vi "Creer un profil EUROTHERM EPC3000.vi"() -> ()   [LabVIEW 2022 SP3]
uses:
  Enum/Enum r15.ctl
  <vilib>/Utility/miscctls.llb/LVDateTimeRec.ctl
  Variables globales/Variable glob generale.vi
  Variables globales/Variables glob EUROTHERM.vi
panel:
  out "Programme 10":cluster{"chaîne":string, "Valeur":dbl}[][](array[cluster]) {"Valeur" format="%#.2f"}
  out "Programme 9":cluster{"chaîne":string, "Valeur":dbl}[][](array[cluster]) {"Valeur" format="%#.2f"}
  out "Programme 8":cluster{"chaîne":string, "Valeur":dbl}[][](array[cluster]) {"Valeur" format="%#.2f"}
  out "Programme 7":cluster{"chaîne":string, "Valeur":dbl}[][](array[cluster]) {"Valeur" format="%#.2f"}
  out "Programme 6":cluster{"chaîne":string, "Valeur":dbl}[][](array[cluster]) {"Valeur" format="%#.2f"}
  out "Programme 5":cluster{"chaîne":string, "Valeur":dbl}[][](array[cluster]) {"Valeur" format="%#.2f"}
  out "référence en sortie":refnum<vi>
  out "Programme 1":cluster{"chaîne":string, "Valeur":dbl}[][](array[cluster]) {"Valeur" format="%#.2f"}
  in  "Insérer segment":bool
  in  "Segment à éditer/supprimer":u8=1 max=26 step=1
  in  "Supprimer segment":bool
  in  "Modif seg":bool
  in  "Charger":bool
  in  "Sauvegarder":bool
  in  "Début du profil":timestamp format="%<%H:%M:%S\n%A %d/%m/%y>T"
  in  "Onglet_Tinit":enum32{"Définir Tinit", "Acquérir Tinit"}(tab)
  in  "Val_Tinit":dbl caption="Valeur initiale. (°C)" format="%.1f"
  in  "Num_reg":u8=1 caption="Adresse régulateur" max=3
  in  "COM régulateur":u16(ring) items=["COM2"]
  in  "Ajouter données":bool
  in  "Ajouter segment":bool
  in  "stop":bool
  in  "Visualiser le profil":bool
  in  "A2":bool
  in  "A1":bool
  in  "Palier":bool
  in  "RT":bool
  in  "RV":bool
  in  "Fin":bool
  in  "Appel":bool
  in  "Saut":bool
  out "Profil":cluster{"Y":dbl[], "Y":dbl[]}[](graph)
  out "Type de fin":string
  in  "Alarme haute":dbl caption="Alarme haute (°C)" min=-199.9 max=300.0 format="%#.1f"
  in  "Alarme basse":dbl caption="Alarme basse (°C)" min=-199.9 max=300.0 format="%#.1f"
  out "Indicateur_Données à éditer":bool
  in  "Comm_Unité de palier":u16(ring) caption="Unité de palier" items=["Seconde(s)", "Minute(s)", "Heure(s)"]
  in  "Comm_Unité de rampe":u16(ring) caption="Unité de rampe" items=["Seconde(s)", "Minute(s)", "Heure(s)"]
  out "Configuration":cluster{"Command (PV)":string, dbl}[](array[cluster]) {"?" format="%#.2f"}
  out "Programme 4":cluster{"chaîne":string, "Valeur":dbl}[][](array[cluster]) {"Valeur" format="%#.2f"}
  out "Programme 3":cluster{"chaîne":string, "Valeur":dbl}[][](array[cluster]) {"Valeur" format="%#.2f"}
  out "Programme 2":cluster{"chaîne":string, "Valeur":dbl}[][](array[cluster]) {"Valeur" format="%#.2f"}
  in  "Onglets_programmes":T1(tab)
  out "Listing programme 1":string
  out "Listing programme 2":string
  out "Listing programme 3":string
  out "Listing programme 4":string
  out "Listing programme 5":string
  out "Listing programme 6":string
  out "Listing programme 7":string
  out "Listing programme 8":string
  out "Listing programme 9":string
  out "Listing programme 10":string
  in  "Onglet_segments":T2(tab)
  in  "Type de fin":u8(ring) items=["Palier"]
  in  "Pente rampe vitesse":sgl min=0 format="%.1g"
  in  "Cible rampe vitesse":dbl caption="Cible rampe vitesse (°C)" min=-199.9 max=300.0 format="%.1f"
  out "Indicateur_Unité de rampe 2":string
  out "Indicateur_Unité de rampe 1":string
  in  "Durée rampe temps":sgl min=0 format="%.1g"
  in  "Cible rampe temps":dbl caption="Cible rampe temps (°C)" min=-199.9 max=300.0 format="%.1f"
  in  "Durée palier":sgl min=0 format="%.1f"
  out "Indicateur_Unité de palier":string
  in  "Cible saut (°C)":dbl min=-199.9 max=300.0 format="%#.1f"
  in  "Nb cycles":u8 caption="Nombre de cycles"
  in  "Numéro prog":u8=1 caption="Numéro de programme" min=1 max=10
  # "création d'un fichier\ncontenant le profil de régulation EPC3000"
  # "Indice seg.:"
  # "Ce logiciel et les informations qu'il contient, sont la propriété de l’IAS et ne peuvent être diffusés sans l’autorisation de la Station d’étalonnage"
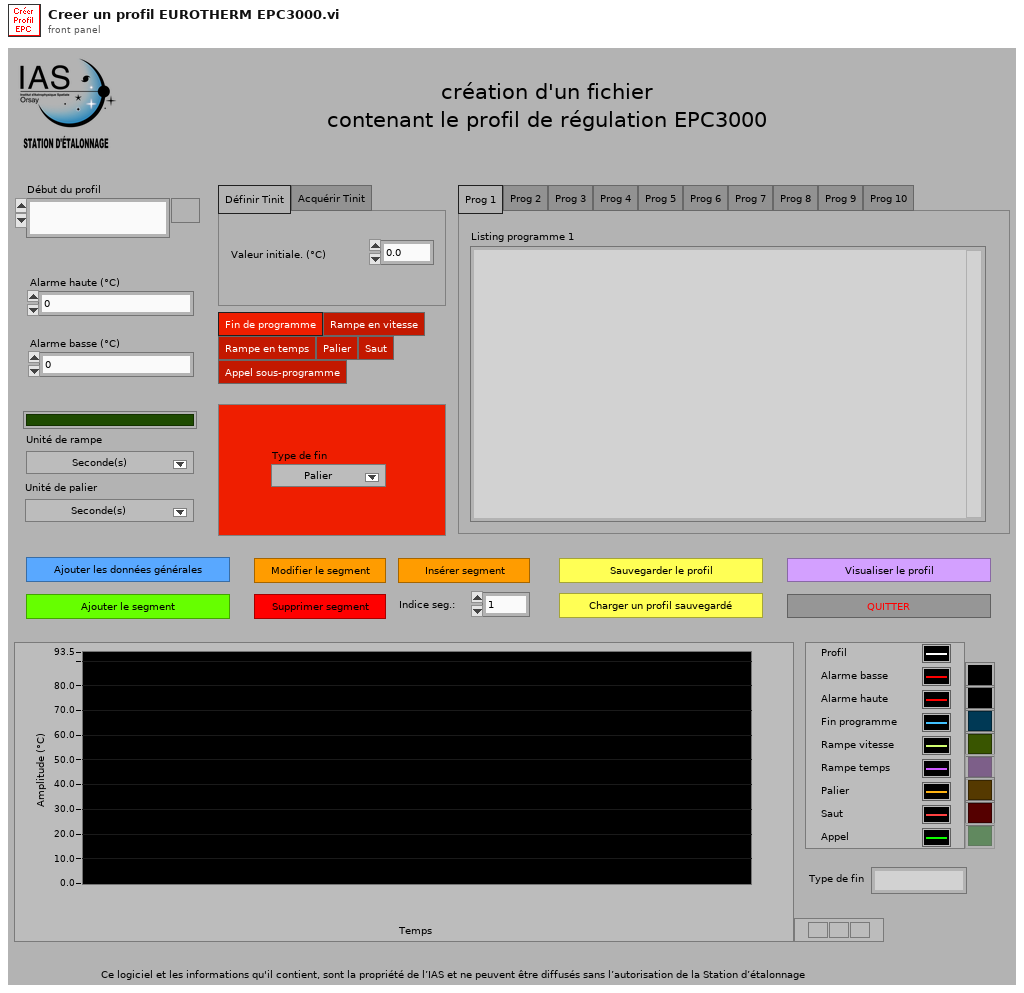
[diagram p1: front panel]
types:
  T1 = enum32{"Prog 1", "Prog 2", "Prog 3", "Prog 4", "Prog 5", "Prog 6", "Prog 7", "Prog 8", "Prog 9", "Prog 10"}
  T2 = enum32{"Fin de programme", "Rampe en vitesse", "Rampe en temps", "Palier", "Saut", "Appel sous-programme"}
  T3 = enum32{"Invalid", "Standard", "Closed", "Hidden", "Minimized", "Maximized"}
  T4 = typedef "Enum r15.ctl" = enum16{"init", "ouvrir fichier", "config", "prog 1", "prog 2", "prog 3", "prog 4", "prog 5", "prog 6", "prog 7", "prog 8", "prog 9", "prog 10", "fin"}
  T5 = cluster{"config":cluster{"key":string, "value":dbl}[], "Prog 1":cluster{string, dbl}[][], "Prog 2":cluster{string, dbl}[][], "Prog 3":cluster{string, dbl}[][], "Prog 4":cluster{string, dbl}[][], "Prog 5":cluster{string, dbl}[][], "Prog 6":cluster{string, dbl}[][], "Prog 7":cluster{string, dbl}[][], "Prog 8":cluster{string, dbl}[][], "Prog 9":cluster{string, dbl}[][], "Prog 10":cluster{string, dbl}[][]}
  T6 = typedef "LVDateTimeRec.ctl" = cluster{"fractional second":dbl, "second":i32, "minute":i32, "hour":i32, "day of month":i32, "month":i32, "year":i32, "day of week":i32, "day of year":i32, "DST":i32}
  T7 = cluster{"chaîne o":string, "Received Value":dbl}[][]
  T8 = cluster{"Configuration":cluster{"Command (PV)":string, dbl}[], "Programme_sortie":cluster{"chaîne":string, "Valeur":dbl}[][], "Programme_sortie":cluster{"chaîne":string, "Valeur":dbl}[][], "Programme_sortie":cluster{"chaîne":string, "Valeur":dbl}[][], "Programme_sortie":cluster{"chaîne":string, "Valeur":dbl}[][], "Programme_sortie":cluster{"chaîne":string, "Valeur":dbl}[][], "Programme_sortie":cluster{"chaîne":string, "Valeur":dbl}[][], "Programme_sortie":cluster{"chaîne":string, "Valeur":dbl}[][], "Programme_sortie":cluster{"chaîne":string, "Valeur":dbl}[][], "Programme_sortie":cluster{"chaîne":string, "Valeur":dbl}[][], "Programme_sortie":cluster{"chaîne":string, "Valeur":dbl}[][]}
  T9 = enum8{"Enabled", "Disabled", "Disabled and Grayed Out"}
  T10 = cluster{"Configuration":cluster{"Command (PV)":string, dbl}[], "Programme 1":cluster{"chaîne":string, "Valeur":dbl}[][], "Programme 2":cluster{"chaîne":string, "Valeur":dbl}[][], "Programme 3":cluster{"chaîne":string, "Valeur":dbl}[][], "Programme 4":cluster{"chaîne":string, "Valeur":dbl}[][], "Programme 5":cluster{"chaîne":string, "Valeur":dbl}[][], "Programme 6":cluster{"chaîne":string, "Valeur":dbl}[][], "Programme 7":cluster{"chaîne":string, "Valeur":dbl}[][], "Programme 8":cluster{"chaîne":string, "Valeur":dbl}[][], "Programme 9":cluster{"chaîne":string, "Valeur":dbl}[][], "Programme 10":cluster{"chaîne":string, "Valeur":dbl}[][]}
  T11 = cluster{"Ev_Saut":dbl[], "Ev_Palier":dbl[], "Ev_Rampe_vitesse":dbl[], "Ev_Rampe_temps":dbl[], "Ev_Appel":dbl[], "Ev_Fin":dbl[], "T_Fin":dbl[], "T_Appel":dbl[], "T_Rampe_temps":dbl[], "T_Rampe_vitesse":dbl[], "T_Palier":dbl[], "T_Saut":dbl[], "Type de fin":string}
  T12 = cluster{"Tempé. max":dbl, "Tempé. min":dbl, "Temps max":dbl, "Temps min":dbl}
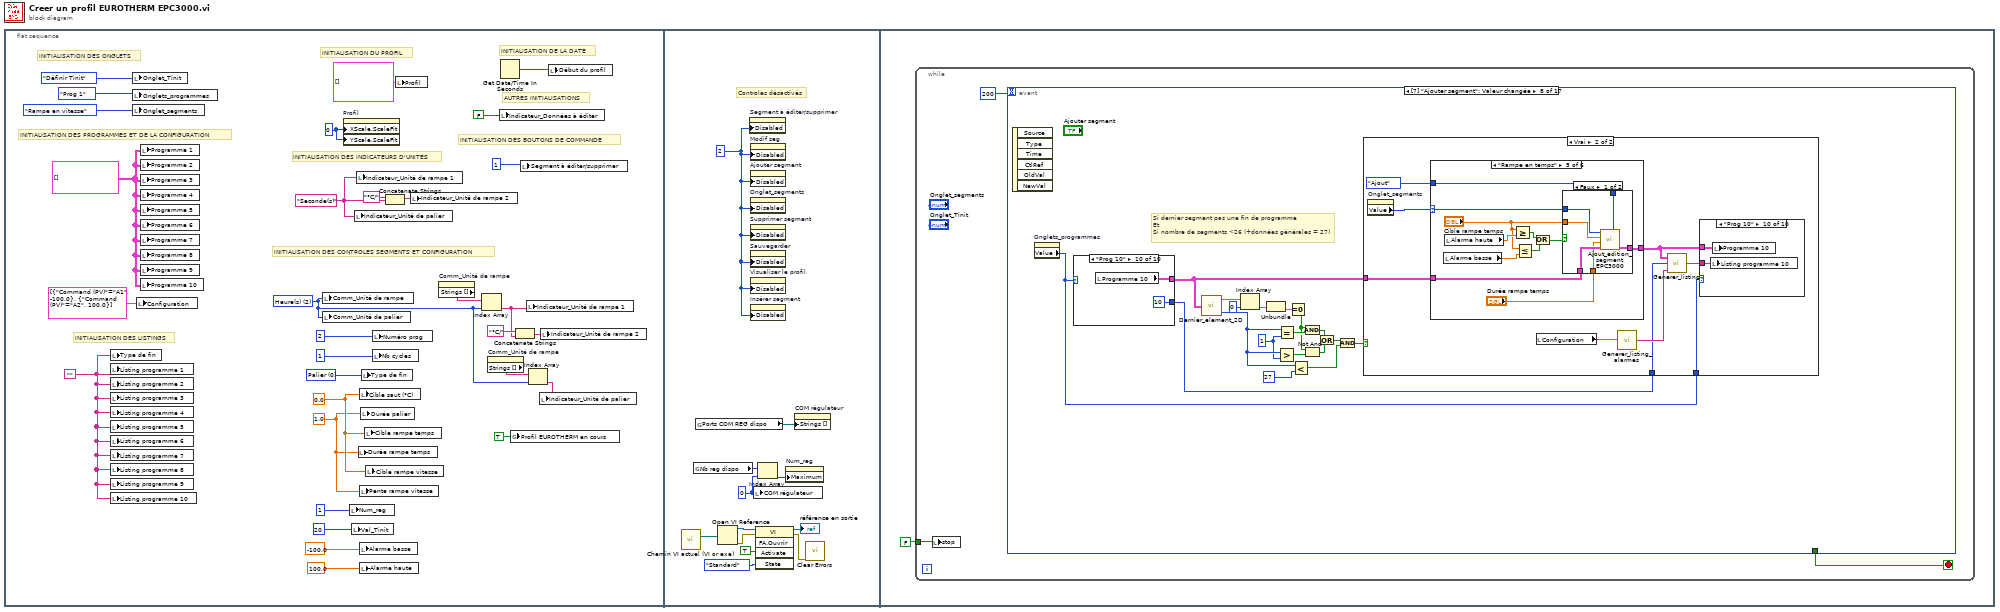
[diagram p0: block diagram]
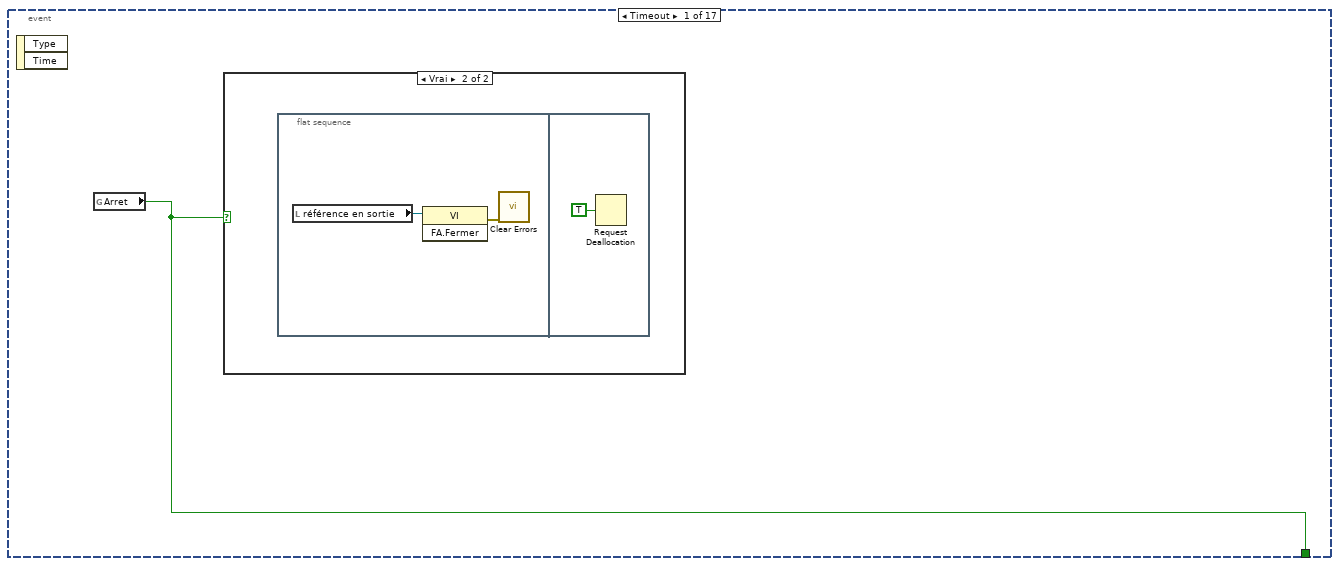
[diagram p2: hidden frame]
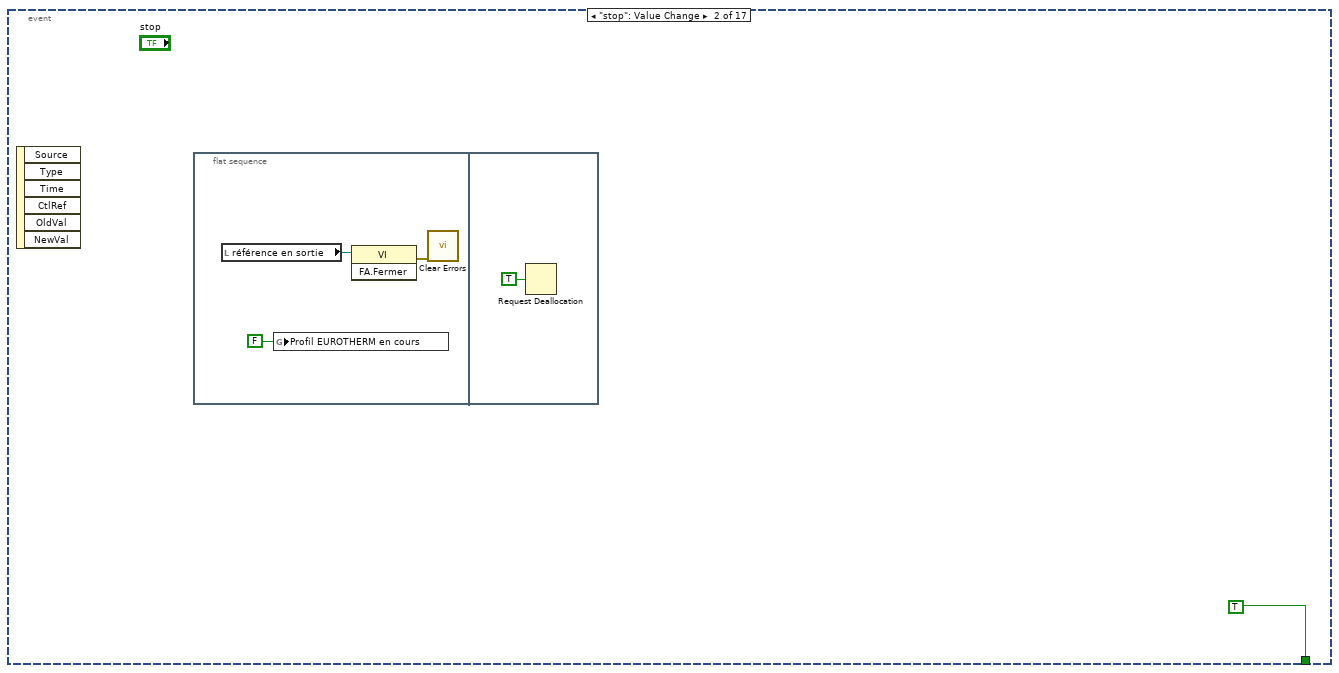
[diagram p4: hidden frame]
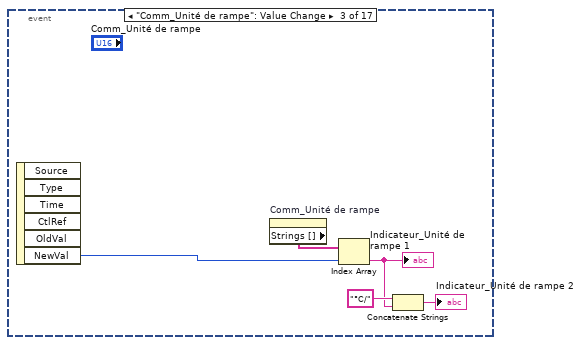
[diagram p5: hidden frame]
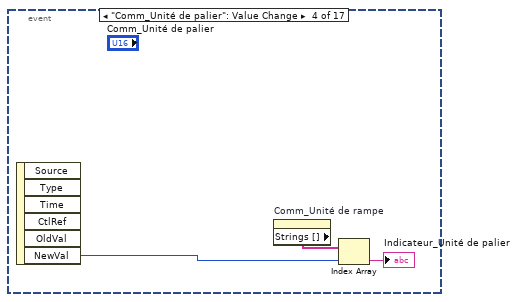
[diagram p6: hidden frame]
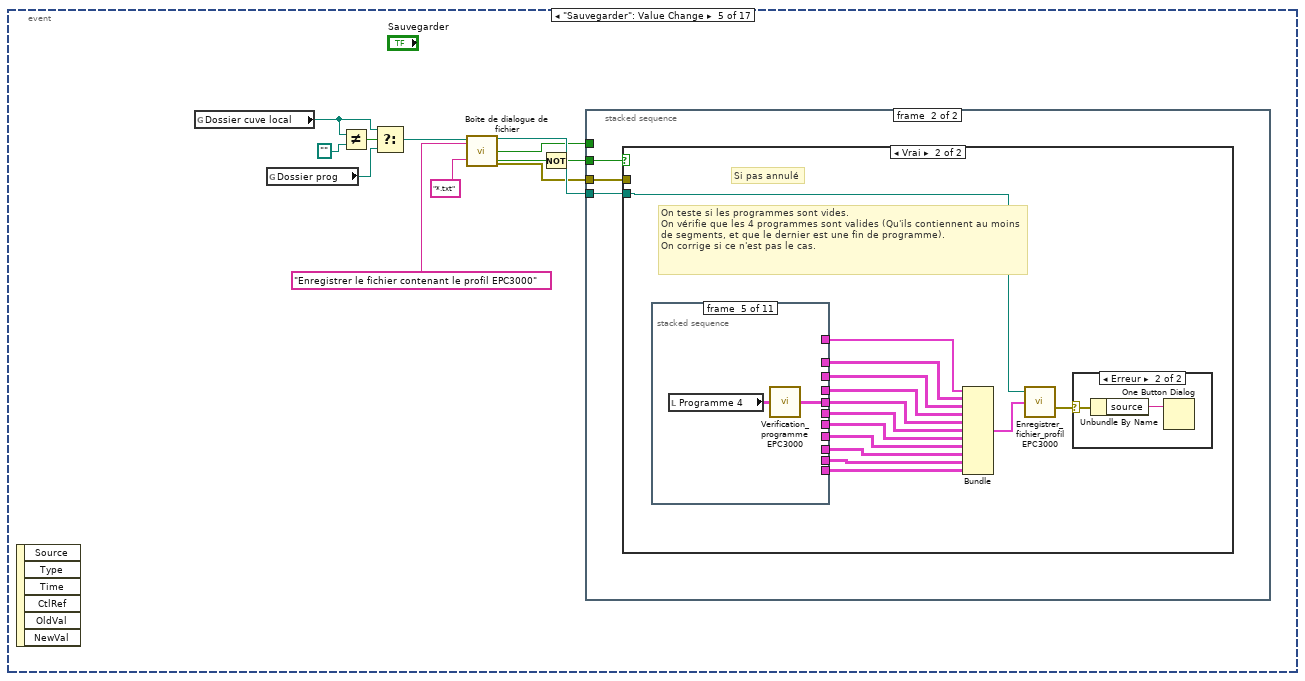
[diagram p7: hidden frame]
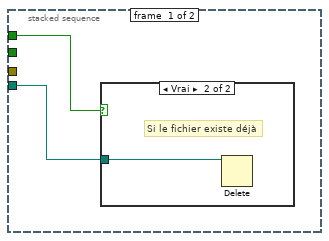
[diagram p8: hidden frame]
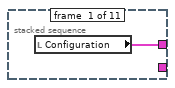
[diagram p11: hidden frame]
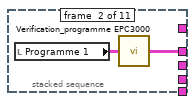
[diagram p12: hidden frame]
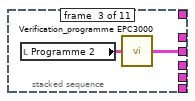
[diagram p13: hidden frame]
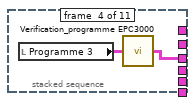
[diagram p14: hidden frame]
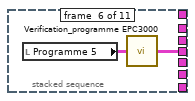
[diagram p15: hidden frame]
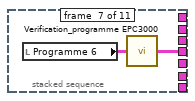
[diagram p16: hidden frame]
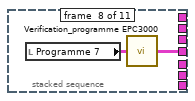
[diagram p17: hidden frame]
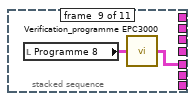
[diagram p18: hidden frame]
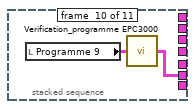
[diagram p19: hidden frame]
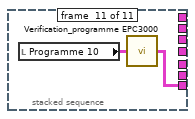
[diagram p20: hidden frame]
diagram:
  n1 = flat-sequence {
    frame #0 {
      w11 = u8 0 items=["Palier"] ("Comm_Type de fin")
      w17 = 1.0 ("Durée rampe temps")
      w18 = 0.0 ("Cible saut (°C)")
      w4 = u16 2 items=["Seconde(s)", "Minute(s)", "Heure(s)"] ("Unité de rampe")
      w23 = u8 0 ("Échelle des X.Ajuster l'échelle")
      w1 = ""
      w2 = T7 [] ("Programme 1")
      w28 = "Seconde(s)" ("Unité de rampe 1")
      # "INITIALISATION DES CONTROLES SEGMENTS ET CONFIGURATION"
      # "AUTRES INITIALISATIONS"
      # "INITIALISATION DES BOUTONS DE COMMANDE"
      # "INITIALISATION DU PROFIL"
      # "INITIALISATION DES LISTINGS"
      # "INITIALISATION DES PROGRAMMES ET DE LA CONFIGURATION"
      # "INITIALISATION DES INDICATEURS D'UNITES"
      # "INITIALISATION DE LA DATE"
      # "INITIALISATION DES ONGLETS"
      n2 = local write "Type de fin"(w1) -> ()
      n3 = local write "Listing programme 1"(w1) -> ()
      n4 = local write "Listing programme 2"(w1) -> ()
      n5 = local write "Listing programme 3"(w1) -> ()
      n6 = local write "Listing programme 4"(w1) -> ()
      n7 = local write "Listing programme 5"(w1) -> ()
      n8 = local write "Listing programme 6"(w1) -> ()
      n9 = local write "Listing programme 7"(w1) -> ()
      n10 = local write "Listing programme 8"(w1) -> ()
      n11 = local write "Listing programme 9"(w1) -> ()
      n12 = local write "Listing programme 10"(w1) -> ()
      n13 = local write "Onglet_Tinit"(enum32{"Définir Tinit", "Acquérir Tinit"}."Définir Tinit" ("Onglet_Tinit")) -> ()
      n14 = local write "Onglets_programmes"(T1."Prog 1" ("Onglets_programmes")) -> ()
      n15 = local write "Onglet_segments"(T2."Rampe en vitesse" ("Commande onglet")) -> ()
      n16 = local write "Configuration"(cluster{"Command (PV)":string, dbl}[] [{"Command (PV)"="A1", -100.0}, {"Command (PV)"="A2", 100.0}] ("Configuration")) -> ()
      n17 = local write "Programme 1"(w2) -> ()
      n18 = local write "Programme 2"(w2) -> ()
      n19 = local write "Programme 3"(w2) -> ()
      n20 = local write "Programme 4"(w2) -> ()
      n21 = local write "Programme 5"(w2) -> ()
      n22 = local write "Programme 6"(w2) -> ()
      n23 = local write "Programme 7"(w2) -> ()
      n24 = local write "Programme 8"(w2) -> ()
      n25 = local write "Programme 9"(w2) -> ()
      n26 = local write "Programme 10"(w2) -> ()
      n27 = local write "Comm_Unité de rampe"(w4) -> ()
      n28 = local write "Comm_Unité de palier"(w4) -> ()
      n29 = property on="Profil" class="GraphXY (strict)"("XScale.ScaleFit"=w23, "YScale.ScaleFit"=w23) -> ()  [unwired: 2 in, 2 out]
      n30 = local write "Num_reg"(u16 1 ("Num_reg")) -> ()
      n31 = local write "Val_Tinit"(u16 20 ("Val_Tinit")) -> ()
      n32 = local write "Indicateur_Unité de palier"(w28) -> ()
      n33 = local write "Indicateur_Unité de rampe 1"(w28) -> ()
      n34 = local write "Durée rampe temps"(w17) -> ()
      n35 = local write "Cible saut (°C)"(w18) -> ()
      n36 = local write "Pente rampe vitesse"(w17) -> ()
      n37 = local write "Alarme basse"(-100.0 ("Comm_Alarme basse")) -> ()
      n38 = local write "Alarme haute"(100.0 ("Comm_Alarme basse")) -> ()
      n39 = local write "Durée palier"(w17) -> ()
      n40 = local write "Type de fin"(w11) -> ()
      n41 = local write "Cible rampe temps"(w18) -> ()
      n42 = local write "Cible rampe vitesse"(w18) -> ()
      n43 = local write "Nb cycles"(u8 1 ("Nombre de cycles")) -> ()
      n44 = local write "Numéro prog"(u8 2 ("Numéro de programme")) -> ()
      n45 = Concatenate Strings("°C/" ("chaîne"), w28) -> (w27:string)
      n46 = local write "Profil"(cluster{"Y":dbl[], "Y":dbl[]}[] [] ("Profil")) -> ()
      n47 = local write "Indicateur_Unité de rampe 2"(w27) -> ()
      n48 = property on="Comm_Unité de rampe" class="MDér (strict)"() -> ("Strings []"=w10:string[])  [unwired: 2 in, 2 out]
      n49 = Index Array(array=w10, index=w4) -> (element=w8:string)
      n50 = property on="Comm_Unité de rampe" class="MDér (strict)"() -> ("Strings []"=w6:string[])  [unwired: 2 in, 2 out]
      n51 = local write "Indicateur_Données à éditer"(FALSE ("Indicateur_Données à éditer")) -> ()
      n52 = Get Date/Time In Seconds() -> (seconds since 1Jan1904=w29:timestamp)
      n53 = global write "Variable glob generale.vi" "Profil EUROTHERM en cours"(TRUE ("Profil en cours")) -> ()
      n54 = Concatenate Strings("°C/" ("chaîne"), w8) -> (w7:string)
      n55 = local write "Segment à éditer/supprimer"(u8 1 ("Segment à éditer")) -> ()
      n56 = local write "Indicateur_Unité de rampe 1"(w8) -> ()
      n57 = Index Array(array=w6, index=w4) -> (element=w5:string)
      n58 = local write "Indicateur_Unité de palier"(w5) -> ()
      n59 = local write "Indicateur_Unité de rampe 2"(w7) -> ()
      n60 = local write "Début du profil"(w29) -> ()
    }
    frame #1 {
      w32 = u16 0
      w43 = u8 2 ("Désactivé")
      # "Controles désactivés"
      n61 = call "Chemin VI actuel (VI or exe).vi"() -> ("Full Path to VI or executable"=w36:path)  [unwired: 14 in, 1 out]
      n62 = global read "Variables glob EUROTHERM.vi" "Nb reg dispo"() -> (w34:u8[])
      n63 = global read "Variables glob EUROTHERM.vi" "Ports COM REG dispo"() -> (w35:refnum<visa-resource-name>[])
      n64 = Open VI Reference(vi path=w36) -> (vi reference=w40:refnum<vi>, error out=w38:errorcluster)  [unwired: 5 in]
      n65 = property on="Segment à éditer/supprimer" class="NumNb (strict)"("Disabled"=w43) -> ()  [unwired: 2 in, 2 out]
      n66 = property on="Modif seg" class="Bool"("Disabled"=w43) -> ()  [unwired: 2 in, 2 out]
      n67 = property on="Ajouter segment" class="Bool"("Disabled"=w43) -> ()  [unwired: 2 in, 2 out]
      n68 = property on="Onglet_segments" class="Onglet (strict)"("Disabled"=w43) -> ()  [unwired: 2 in, 2 out]
      n69 = property on="Supprimer segment" class="Bool"("Disabled"=w43) -> ()  [unwired: 2 in, 2 out]
      n70 = property on="Sauvegarder" class="Bool"("Disabled"=w43) -> ()  [unwired: 2 in, 2 out]
      n71 = property on="Visualiser le profil" class="Bool"("Disabled"=w43) -> ()  [unwired: 2 in, 2 out]
      n72 = property on="Insérer segment" class="Bool"("Disabled"=w43) -> ()  [unwired: 2 in, 2 out]
      n73 = local write "COM régulateur"(w32) -> ()
      n74 = invoke class="VI" method="FA.Ouvrir"(reference=w40, error in=w38, "Activate"=TRUE ("Activer ?"), "State"=T3."Standard" ("État")) -> (reference out=→"référence en sortie":refnum<vi>, error out=w37:errorcluster)  [unwired: 1 in, 3 out]
      n75 = Index Array(array=w34, index=w32) -> (element=w33:u8)
      n76 = property on="Num_reg" class="NumNb (strict)"("Maximum"=w33) -> ()  [unwired: 2 in, 2 out]
      n77 = property on="COM régulateur" class="MDér (strict)"("Strings []"=w35) -> ()  [unwired: 2 in, 2 out]
      n78 = call <vilib>:"Clear Errors.vi"("error in (no error)"=w37) -> ()  [unwired: 5 in, 2 out]
    }
    frame #2 {
      n79 = while {
        tunnel: FALSE ("stop") -> [w46]
        stop <- w47 stop-if-true
        n80 = local write "stop"(w46) -> ()
        n81 = event shown="[7] \"Ajouter segment\": Valeur changée" {
          selector: _ -> [_ _ _ _ _ _ _ _ _ _ _ _ _ _ _ _ _]
          dyn-events: _ -> [_ _ _ _ _ _ _ _ _ _ _ _ _ _ _ _ _]
          timeout: 200 -> [_ _ _ _ _ _ _ _ _ _ _ _ _ _ _ _ _]
          tunnel: [w48 TRUE ("stop") _ _ _ _ _ _ _ _ _ _ _ _ _ _ _] -> w47
          event Timeout {
            n82 = event-data() -> ()  [unwired: 1 in, 2 out]
            n83 = global read "Variable glob generale.vi" "Arret"() -> (w48:bool)
            n84 = case shown="Vrai" w48 {
              frame False {
              }
              frame True {
                n85 = flat-sequence {
                  frame #0 {
                    n86 = local read "référence en sortie"() -> (w49:refnum<vi>)
                    n87 = invoke class="VI" method="FA.Fermer"(reference=w49) -> (error out=w50:errorcluster)  [unwired: 2 in, 2 out]
                    n88 = call <vilib>:"Clear Errors.vi"("error in (no error)"=w50) -> ()  [unwired: 5 in, 2 out]
                  }
                  frame #1 {
                    n89 = Request Deallocation(TRUE ("flag")) -> ()
                  }
                }
              }
            }
          }
          event "stop": Value Change {
            n90 = event-data() -> ()  [unwired: 1 in, 6 out]
            n91 = flat-sequence {
              frame #0 {
                n92 = local read "référence en sortie"() -> (w54:refnum<vi>)
                n93 = global write "Variable glob generale.vi" "Profil EUROTHERM en cours"(FALSE ("Profil en cours")) -> ()
                n94 = invoke class="VI" method="FA.Fermer"(reference=w54) -> (error out=w55:errorcluster)  [unwired: 2 in, 2 out]
                n95 = call <vilib>:"Clear Errors.vi"("error in (no error)"=w55) -> ()  [unwired: 5 in, 2 out]
              }
              frame #1 {
                n96 = Request Deallocation(TRUE ("flag")) -> ()
              }
            }
          }
          event "Comm_Unité de rampe": Value Change {
            n97 = event-data() -> ("NewVal"=w60:u16)  [unwired: 1 in, 5 out]
            n98 = property on="Comm_Unité de rampe" class="MDér (strict)"() -> ("Strings []"=w61:string[])  [unwired: 2 in, 2 out]
            n99 = Index Array(array=w61, index=w60) -> (element=w58:string)
            "Indicateur_Unité de rampe 1" <- w58
            n100 = Concatenate Strings("°C/" ("chaîne"), w58) -> (→"Indicateur_Unité de rampe 2":string)
          }
          event "Comm_Unité de palier": Value Change {
            n101 = event-data() -> ("NewVal"=w63:u16)  [unwired: 1 in, 5 out]
            n102 = property on="Comm_Unité de rampe" class="MDér (strict)"() -> ("Strings []"=w64:string[])  [unwired: 2 in, 2 out]
            n103 = Index Array(array=w64, index=w63) -> (element=→"Indicateur_Unité de palier":string)
          }
          event "Sauvegarder": Value Change {
            n104 = event-data() -> ()  [unwired: 1 in, 6 out]
            n105 = global read "Variable glob generale.vi" "Dossier cuve local"() -> (w67:path)
            n106 = global read "Variable glob generale.vi" "Dossier prog"() -> (w66:path)
            n107 = Not Equal?(x=w67, y=path "") -> (x != y?=w68:bool)
            n108 = Select(t=w67, s=w68, f=w66) -> (s? t:f=w65:path)
            n109 = call "Boîte de dialogue de fichier"("start path"=w65, "prompt"="Enregistrer le fichier contenant le profil EPC3000", "pattern (all files)"="*.txt") -> ("selected path"=w76:path, "exists"=w71:bool, "cancelled"=w74:bool, "error out"=w72:errorcluster)  [unwired: 9 in]
            n110 = Not(x=w74) -> (.not. x?=w73:bool)
            n111 = stacked-sequence {
              tunnel: w76 -> [w77 w82]
              tunnel: w73 -> [_ w81]
              tunnel: w72 -> [_ w80]
              tunnel: w71 -> [w78 _]
              frame #0 {
                n112 = case shown="Vrai" w78 {
                  tunnel: w77 -> [_ w79]
                  frame False {
                  }
                  frame True {
                    # "Si le fichier existe déjà"
                    n113 = Delete(path (use dialog)=w79) -> ()  [unwired: 4 in, 3 out]
                  }
                }
              }
              frame #1 {
                n114 = case shown="Vrai" w81 {
                  tunnel: w82 -> [_ w96]
                  tunnel: w80 -> [_ _]
                  frame False {
                  }
                  frame True {
                    # "On teste si les programmes sont vides. \nOn vérifie que les 4 programmes sont valides (Qu'ils contiennent au moins de segments, et que le dernier est une fin de programme).\nOn corrige si ce n'est pas le cas."
                    # "Si pas annulé"
                    n115 = stacked-sequence {
                      tunnel: [w97 _ _ _ _ _ _ _ _ _ _] -> w93
                      tunnel: [_ w98 _ _ _ _ _ _ _ _ _] -> w92
                      tunnel: [_ _ w100 _ _ _ _ _ _ _ _] -> w91
                      tunnel: [_ _ _ w102 _ _ _ _ _ _ _] -> w90
                      tunnel: [_ _ _ _ w104 _ _ _ _ _ _] -> w89
                      tunnel: [_ _ _ _ _ w106 _ _ _ _ _] -> w88
                      tunnel: [_ _ _ _ _ _ w108 _ _ _ _] -> w87
                      tunnel: [_ _ _ _ _ _ _ w110 _ _ _] -> w86
                      tunnel: [_ _ _ _ _ _ _ _ w112 _ _] -> w85
                      tunnel: [_ _ _ _ _ _ _ _ _ w114 _] -> w84
                      tunnel: [_ _ _ _ _ _ _ _ _ _ w116] -> w83
                      frame #0 {
                        n116 = local read "Configuration"() -> (w97:cluster{"Command (PV)":string, dbl}[])
                      }
                      frame #1 {
                        n117 = local read "Programme 1"() -> (w99:cluster{"chaîne":string, "Valeur":dbl}[][])
                        n118 = call "Verification_programme EPC3000.vi"("Programme_entrée"=w99) -> ("Programme_sortie"=w98:cluster{"chaîne":string, "Valeur":dbl}[][])
                      }
                      frame #2 {
                        n119 = local read "Programme 2"() -> (w101:cluster{"chaîne":string, "Valeur":dbl}[][])
                        n120 = call "Verification_programme EPC3000.vi"("Programme_entrée"=w101) -> ("Programme_sortie"=w100:cluster{"chaîne":string, "Valeur":dbl}[][])
                      }
                      frame #3 {
                        n121 = local read "Programme 3"() -> (w103:cluster{"chaîne":string, "Valeur":dbl}[][])
                        n122 = call "Verification_programme EPC3000.vi"("Programme_entrée"=w103) -> ("Programme_sortie"=w102:cluster{"chaîne":string, "Valeur":dbl}[][])
                      }
                      frame #4 {
                        n123 = local read "Programme 4"() -> (w105:cluster{"chaîne":string, "Valeur":dbl}[][])
                        n124 = call "Verification_programme EPC3000.vi"("Programme_entrée"=w105) -> ("Programme_sortie"=w104:cluster{"chaîne":string, "Valeur":dbl}[][])
                      }
                      frame #5 {
                        n125 = local read "Programme 5"() -> (w107:cluster{"chaîne":string, "Valeur":dbl}[][])
                        n126 = call "Verification_programme EPC3000.vi"("Programme_entrée"=w107) -> ("Programme_sortie"=w106:cluster{"chaîne":string, "Valeur":dbl}[][])
                      }
                      frame #6 {
                        n127 = local read "Programme 6"() -> (w109:cluster{"chaîne":string, "Valeur":dbl}[][])
                        n128 = call "Verification_programme EPC3000.vi"("Programme_entrée"=w109) -> ("Programme_sortie"=w108:cluster{"chaîne":string, "Valeur":dbl}[][])
                      }
                      frame #7 {
                        n129 = local read "Programme 7"() -> (w111:cluster{"chaîne":string, "Valeur":dbl}[][])
                        n130 = call "Verification_programme EPC3000.vi"("Programme_entrée"=w111) -> ("Programme_sortie"=w110:cluster{"chaîne":string, "Valeur":dbl}[][])
                      }
                      frame #8 {
                        n131 = local read "Programme 8"() -> (w113:cluster{"chaîne":string, "Valeur":dbl}[][])
                        n132 = call "Verification_programme EPC3000.vi"("Programme_entrée"=w113) -> ("Programme_sortie"=w112:cluster{"chaîne":string, "Valeur":dbl}[][])
                      }
                      frame #9 {
                        n133 = local read "Programme 9"() -> (w115:cluster{"chaîne":string, "Valeur":dbl}[][])
                        n134 = call "Verification_programme EPC3000.vi"("Programme_entrée"=w115) -> ("Programme_sortie"=w114:cluster{"chaîne":string, "Valeur":dbl}[][])
                      }
                      frame #10 {
                        n135 = local read "Programme 10"() -> (w117:cluster{"chaîne":string, "Valeur":dbl}[][])
                        n136 = call "Verification_programme EPC3000.vi"("Programme_entrée"=w117) -> ("Programme_sortie"=w116:cluster{"chaîne":string, "Valeur":dbl}[][])
                      }
                    }
                    n137 = Bundle("Configuration"=w93, "Programme_sortie"=w92, "Programme_sortie"=w91, "Programme_sortie"=w90, "Programme_sortie"=w89, "Programme_sortie"=w88, "Programme_sortie"=w87, "Programme_sortie"=w86, "Programme_sortie"=w85, "Programme_sortie"=w84, "Programme_sortie"=w83) -> (w95:T8)  [unwired: 1 in]
                    n138 = call "Enregistrer_fichier_profil EPC3000.vi"("Config + programmes"=w95, "Chemin du fichier profil"=w96) -> ("error out 2"=w94:errorcluster)  [unwired: 1 in, 1 out]
                    n139 = case shown="Erreur" w94 {
                      selector: w94 -> [_ w119]
                      frame No Error {
                      }
                      frame Error {
                        n140 = Unbundle By Name(w119) -> ("source"=w118:string)
                        n141 = One Button Dialog(message=w118) -> ()  [unwired: 1 in, 1 out]
                      }
                    }
                  }
                }
              }
            }
          }
          event "Charger": Value Change {
            # "On teste si les programmes sont vides. \nOn vérifie que les 4 programmes sont valides (Qu'ils contiennent au moins de segments, et que le dernier est une fin de programme).\nOn corrige si ce n'est pas le cas."
            n142 = event-data() -> ()  [unwired: 1 in, 6 out]
            n143 = while {
              shift-right: [w128] -> _
              shift-left: Enum_r15."init" ("Énum") -> [w129]
              shift-right: [w127] -> _
              shift-left: _ -> [w126]
              shift-right: [w125] -> _
              shift-left: _ -> [w124]
              stop <- w123 stop-if-true
              n144 = case shown="\"init\", Par défaut" w129 {
                tunnel: [Enum_r15."ouvrir fichier" ("Énum") w156 Enum_r15."prog 1" ("Énum") Enum_r15."prog 2" ("Énum") Enum_r15."prog 3" ("Énum") Enum_r15."prog 4" ("Énum") Enum_r15."prog 5" ("Énum") Enum_r15."prog 6" ("Énum") Enum_r15."prog 7" ("Énum") Enum_r15."prog 8" ("Énum") Enum_r15."prog 9" ("Énum") Enum_r15."prog 10" ("Énum") Enum_r15."fin" ("Énum") Enum_r15."init" ("Énum")] -> w128
                tunnel: [T5 {"config"=[], "Prog 1"=[], "Prog 2"=[], "Prog 3"=[], "Prog 4"=[], "Prog 5"=[], "Prog 6"=[], "Prog 7"=[], "Prog 8"=[], "Prog 9"=[], "Prog 10"=[]} ("Config + programmes") w154 w178 w188 w204 w211 w218 w225 w232 w239 w246 w253 w260 T5 {"config"=[], "Prog 1"=[], "Prog 2"=[], "Prog 3"=[], "Prog 4"=[], "Prog 5"=[], "Prog 6"=[], "Prog 7"=[], "Prog 8"=[], "Prog 9"=[], "Prog 10"=[]} ("Config + programmes")] -> w127
                tunnel: w126 -> [_ _ w178 w188 w204 w211 w218 w225 w232 w239 w246 w253 w260 _]
                tunnel: ["" ("Listing alarmes") w153 w172 w186 w203 w212 w219 w226 w233 w240 w247 w254 w261 "" ("Listing alarmes")] -> w125
                tunnel: w124 -> [_ w153 _ w186 w203 w212 w219 w226 w233 w240 w247 w254 w261 _]
                tunnel: [_ _ _ _ _ _ _ _ _ _ _ _ _ TRUE] -> w123
                frame "init", Default {
                  w130 = T9."Enabled" ("Désactivé")
                  w134 = u8 0 ("Échelle des X.Ajuster l'échelle")
                  # "Controles activés"
                  # "INITIALISATION DU PROFIL"
                  # "INITIALISATION DE LA DATE"
                  n145 = Get Date/Time In Seconds() -> (seconds since 1Jan1904=w135:timestamp)
                  n146 = local write "Début du profil"(w135) -> ()
                  n147 = property on="Profil" class="GraphXY (strict)"("XScale.ScaleFit"=w134, "YScale.ScaleFit"=w134) -> ()  [unwired: 2 in, 2 out]
                  n148 = local write "Type de fin"("") -> ()
                  n149 = local write "Profil"(cluster{"Y":dbl[], "Y":dbl[]}[] [] ("Profil")) -> ()
                  n150 = property on="Insérer segment" class="Bool"("Disabled"=w130) -> ()  [unwired: 2 in, 2 out]
                  n151 = property on="Modif seg" class="Bool"("Disabled"=w130) -> ()  [unwired: 2 in, 2 out]
                  n152 = property on="Ajouter segment" class="Bool"("Disabled"=w130) -> ()  [unwired: 2 in, 2 out]
                  n153 = property on="Sauvegarder" class="Bool"("Disabled"=w130) -> ()  [unwired: 2 in, 2 out]
                  n154 = property on="Visualiser le profil" class="Bool"("Disabled"=w130) -> ()  [unwired: 2 in, 2 out]
                  n155 = property on="Segment à éditer/supprimer" class="NumNb (strict)"("Disabled"=w130) -> ()  [unwired: 2 in, 2 out]
                  n156 = property on="Onglet_segments" class="Onglet (strict)"("Disabled"=w130) -> ()  [unwired: 2 in, 2 out]
                  n157 = property on="Supprimer segment" class="Bool"("Disabled"=w130) -> ()  [unwired: 2 in, 2 out]
                }
                frame "ouvrir fichier" {
                  n158 = global read "Variable glob generale.vi" "Dossier cuve local"() -> (w148:path)
                  n159 = global read "Variable glob generale.vi" "Dossier prog"() -> (w147:path)
                  n160 = Not Equal?(x=w148, y=path "") -> (x != y?=w149:bool)
                  n161 = Select(t=w148, s=w149, f=w147) -> (s? t:f=w144:path)
                  n162 = Not Equal?(x=w144, y=path "") -> (x != y?=w145:bool)
                  n163 = Select(t=w144, s=w145, f=path "C://Data" ("cas faux")) -> (s? t:f=w142:path)
                  n164 = call "Boîte de dialogue de fichier2"("start path"=w142, "prompt"="Nom du fichier contenant le profil EPC3000", "pattern (all files)"="*.txt") -> ("selected path"=w151:path, "cancelled"=w139:bool, "error out"=w141:errorcluster)  [unwired: 9 in, 1 out]
                  n165 = Unbundle By Name(w141) -> ("status"=w140:bool)
                  n166 = Or(x=w139, y=w140) -> (x .or. y?=w138:bool)
                  n167 = case shown="Faux" w138 {
                    tunnel: w151 -> [w163 _]
                    tunnel: [w162 FALSE] -> w155
                    tunnel: [w161 T5 {"config"=[], "Prog 1"=[], "Prog 2"=[], "Prog 3"=[], "Prog 4"=[], "Prog 5"=[], "Prog 6"=[], "Prog 7"=[], "Prog 8"=[], "Prog 9"=[], "Prog 10"=[]} ("Config + programmes")] -> w154
                    frame False {
                      n168 = call "Lire_fichier_profil EPC3000.vi"("Chemin du fichier profil"=w163) -> ("error out"=w164:errorcluster, "Config + programmes"=w161:T5)  [unwired: 1 in]
                      n169 = case shown="Erreur" w164 {
                        selector: w164 -> [_ w168]
                        tunnel: [TRUE FALSE] -> w162
                        frame No Error {
                        }
                        frame Error {
                          n170 = Unbundle By Name(w168) -> ("source"=w167:string)
                          n171 = One Button Dialog(message=w167) -> ()  [unwired: 1 in, 1 out]
                        }
                      }
                    }
                    frame True {
                      # "annulé"
                    }
                  }
                  n172 = Strip Path(path=w151) -> (stripped path=w152:path)  [unwired: 1 out]
                  n173 = global write "Variable glob generale.vi" "Dossier prog"(w152) -> ()
                  n174 = Select(t=Enum_r15."config" ("Énum"), s=w155, f=Enum_r15."fin" ("Énum")) -> (s? t:f=w156:T4)
                }
                frame "config" {
                  n175 = Unbundle By Name(w178) -> ("config"=w173:cluster{"key":string, "value":dbl}[])
                  "Configuration" <- w173
                  n176 = call "Generer_listing_alarmes.vi"("Configuration"=w173) -> ("Listing alarmes"=w172:string)
                  n177 = Index Array(array=w173) -> (element #1=w174:cluster{"key":string, "value":dbl}, element #2=w177:cluster{"key":string, "value":dbl})  [unwired: 2 in]
                  n178 = Unbundle(w174) -> ("value"=w176:dbl)  [unwired: 1 out]
                  n179 = Unbundle(w177) -> ("value"=w175:dbl)  [unwired: 1 out]
                  n180 = local write "Alarme basse"(w176) -> ()
                  n181 = local write "Alarme haute"(w175) -> ()
                }
                frame "prog 1" {
                  n182 = Unbundle By Name(w188) -> ("Prog 1"=w187:cluster{string, dbl}[][])
                  n183 = call "Verification_programme EPC3000.vi"("Programme_entrée"=w187) -> ("Programme_sortie"=w184:cluster{"chaîne":string, "Valeur":dbl}[][])
                  "Programme 1" <- w184
                  n184 = call "Generer_listing.vi"("Listing_entrée"=w186, "Numéro de programme"=u8 1, "Programme"=w184) -> ("Listing_sortie"=→"Listing programme 1":string)
                  n185 = Index Array(array=w184) -> (element=w192:cluster{"chaîne":string, "Valeur":dbl}[])  [unwired: 2 in]
                  n186 = Index Array(array=w184, index (row)=1 ("indice (ligne)"), index (col)=0 ("indice désactivé (col)")) -> (element=w181:cluster{"chaîne":string, "Valeur":dbl})
                  n187 = Index Array(array=w192) -> (element #1=w191:cluster{"chaîne":string, "Valeur":dbl}, element #2=w190:cluster{"chaîne":string, "Valeur":dbl})  [unwired: 2 in]
                  n188 = Unbundle By Name(w181) -> ("Valeur"=w180:dbl)
                  n189 = Unbundle(w191) -> ("Valeur"=w197:dbl)  [unwired: 1 out]
                  n190 = Unbundle(w190) -> ("Valeur"=w200:dbl)  [unwired: 1 out]
                  n191 = To Unsigned Long Integer(number=w180) -> (unsigned 32bit integer=w179:u32)
                  n192 = property on="Comm_Unité de rampe" class="MDér (strict)"() -> ("Strings []"=w196:string[])  [unwired: 2 in, 2 out]
                  n193 = local write "Comm_Unité de rampe"(w197) -> ()
                  n194 = property on="Comm_Unité de palier" class="MDér (strict)"() -> ("Strings []"=w199:string[])  [unwired: 2 in, 2 out]
                  n195 = local write "Comm_Unité de palier"(w200) -> ()
                  n196 = local write "Onglet_segments"(w179) -> ()
                  n197 = Index Array(array=w196, index=w197) -> (element=w194:string)
                  n198 = Index Array(array=w199, index=w200) -> (element=w198:string)
                  n199 = local write "Indicateur_Unité de rampe 1"(w194) -> ()
                  n200 = Concatenate Strings("°C/" ("chaîne"), w194) -> (w195:string)
                  n201 = local write "Indicateur_Unité de palier"(w198) -> ()
                  n202 = local write "Indicateur_Unité de rampe 2"(w195) -> ()
                }
                frame "prog 2" {
                  n203 = Unbundle By Name(w204) -> ("Prog 2"=w205:cluster{string, dbl}[][])
                  n204 = call "Verification_programme EPC3000.vi"("Programme_entrée"=w205) -> ("Programme_sortie"=w206:cluster{"chaîne":string, "Valeur":dbl}[][])
                  "Programme 2" <- w206
                  n205 = call "Generer_listing.vi"("Listing_entrée"=w203, "Numéro de programme"=u8 2, "Programme"=w206) -> ("Listing_sortie"=→"Listing programme 2":string)
                }
                frame "prog 3" {
                  n206 = Unbundle By Name(w211) -> ("Prog 3"=w210:cluster{string, dbl}[][])
                  n207 = call "Verification_programme EPC3000.vi"("Programme_entrée"=w210) -> ("Programme_sortie"=w213:cluster{"chaîne":string, "Valeur":dbl}[][])
                  "Programme 3" <- w213
                  n208 = call "Generer_listing.vi"("Listing_entrée"=w212, "Numéro de programme"=u8 3, "Programme"=w213) -> ("Listing_sortie"=→"Listing programme 3":string)
                }
                frame "prog 4" {
                  n209 = Unbundle By Name(w218) -> ("Prog 4"=w217:cluster{string, dbl}[][])
                  n210 = call "Verification_programme EPC3000.vi"("Programme_entrée"=w217) -> ("Programme_sortie"=w220:cluster{"chaîne":string, "Valeur":dbl}[][])
                  "Programme 4" <- w220
                  n211 = call "Generer_listing.vi"("Listing_entrée"=w219, "Numéro de programme"=u8 4, "Programme"=w220) -> ("Listing_sortie"=→"Listing programme 4":string)
                }
                frame "prog 5" {
                  n212 = Unbundle By Name(w225) -> ("Prog 5"=w224:cluster{string, dbl}[][])
                  n213 = call "Verification_programme EPC3000.vi"("Programme_entrée"=w224) -> ("Programme_sortie"=w228:cluster{"chaîne":string, "Valeur":dbl}[][])
                  "Programme 5" <- w228
                  n214 = call "Generer_listing.vi"("Listing_entrée"=w226, "Numéro de programme"=u8 5, "Programme"=w228) -> ("Listing_sortie"=→"Listing programme 5":string)
                }
                frame "prog 6" {
                  n215 = Unbundle By Name(w232) -> ("Prog 6"=w231:cluster{string, dbl}[][])
                  n216 = call "Verification_programme EPC3000.vi"("Programme_entrée"=w231) -> ("Programme_sortie"=w235:cluster{"chaîne":string, "Valeur":dbl}[][])
                  "Programme 6" <- w235
                  n217 = call "Generer_listing.vi"("Listing_entrée"=w233, "Numéro de programme"=u8 6, "Programme"=w235) -> ("Listing_sortie"=→"Listing programme 6":string)
                }
                frame "prog 7" {
                  n218 = Unbundle By Name(w239) -> ("Prog 7"=w238:cluster{string, dbl}[][])
                  n219 = call "Verification_programme EPC3000.vi"("Programme_entrée"=w238) -> ("Programme_sortie"=w242:cluster{"chaîne":string, "Valeur":dbl}[][])
                  "Programme 7" <- w242
                  n220 = call "Generer_listing.vi"("Listing_entrée"=w240, "Numéro de programme"=u8 7, "Programme"=w242) -> ("Listing_sortie"=→"Listing programme 7":string)
                }
                frame "prog 8" {
                  n221 = Unbundle By Name(w246) -> ("Prog 8"=w245:cluster{string, dbl}[][])
                  n222 = call "Verification_programme EPC3000.vi"("Programme_entrée"=w245) -> ("Programme_sortie"=w249:cluster{"chaîne":string, "Valeur":dbl}[][])
                  "Programme 8" <- w249
                  n223 = call "Generer_listing.vi"("Listing_entrée"=w247, "Numéro de programme"=u8 8, "Programme"=w249) -> ("Listing_sortie"=→"Listing programme 8":string)
                }
                frame "prog 9" {
                  n224 = Unbundle By Name(w253) -> ("Prog 9"=w252:cluster{string, dbl}[][])
                  n225 = call "Verification_programme EPC3000.vi"("Programme_entrée"=w252) -> ("Programme_sortie"=w256:cluster{"chaîne":string, "Valeur":dbl}[][])
                  "Programme 9" <- w256
                  n226 = call "Generer_listing.vi"("Listing_entrée"=w254, "Numéro de programme"=u8 9, "Programme"=w256) -> ("Listing_sortie"=→"Listing programme 9":string)
                }
                frame "prog 10" {
                  n227 = Unbundle By Name(w260) -> ("Prog 10"=w259:cluster{string, dbl}[][])
                  n228 = call "Verification_programme EPC3000.vi"("Programme_entrée"=w259) -> ("Programme_sortie"=w263:cluster{"chaîne":string, "Valeur":dbl}[][])
                  "Programme 10" <- w263
                  n229 = call "Generer_listing.vi"("Listing_entrée"=w261, "Numéro de programme"=u8 10, "Programme"=w263) -> ("Listing_sortie"=→"Listing programme 10":string)
                }
                frame "fin" {
                }
              }
            }
            n230 = local write "Segment à éditer/supprimer"(u8 1 ("Segment à éditer")) -> ()
            n231 = local write "Onglets_programmes"(T1."Prog 1" ("Onglets_programmes")) -> ()
          }
          event "Ajouter données": Value Change {
            w272 = T9."Enabled" ("Désactivé")
            # "Controles activés"
            # "Si programme vide"
            n232 = event-data() -> ()  [unwired: 1 in, 6 out]
            n233 = property on="Onglets_programmes" class="Onglet (strict)"() -> ("Value"=w269:T1)  [unwired: 2 in, 2 out]
            n234 = case shown="\"Prog 10\"" w269 {
              tunnel: [w276 w278 w280 w282 w284 w286 w288 w290 w292 w294] -> w271
              tunnel: [u8 1 ("Numéro de programme") u8 2 ("Numéro de programme") u8 3 ("Numéro de programme") u8 4 ("Numéro de programme") u8 5 ("Numéro de programme") u8 6 ("Numéro de programme") u8 7 ("Numéro de programme") u8 8 ("Numéro de programme") u8 9 ("Numéro de programme") u8 10 ("Numéro de programme")] -> w270
              frame "Prog 1", Default {
                n235 = local read "Programme 1"() -> (w276:cluster{"chaîne":string, "Valeur":dbl}[][])
              }
              frame "Prog 2" {
                n236 = local read "Programme 2"() -> (w278:cluster{"chaîne":string, "Valeur":dbl}[][])
              }
              frame "Prog 3" {
                n237 = local read "Programme 3"() -> (w280:cluster{"chaîne":string, "Valeur":dbl}[][])
              }
              frame "Prog 4" {
                n238 = local read "Programme 4"() -> (w282:cluster{"chaîne":string, "Valeur":dbl}[][])
              }
              frame "Prog 5" {
                n239 = local read "Programme 5"() -> (w284:cluster{"chaîne":string, "Valeur":dbl}[][])
              }
              frame "Prog 6" {
                n240 = local read "Programme 6"() -> (w286:cluster{"chaîne":string, "Valeur":dbl}[][])
              }
              frame "Prog 7" {
                n241 = local read "Programme 7"() -> (w288:cluster{"chaîne":string, "Valeur":dbl}[][])
              }
              frame "Prog 8" {
                n242 = local read "Programme 8"() -> (w290:cluster{"chaîne":string, "Valeur":dbl}[][])
              }
              frame "Prog 9" {
                n243 = local read "Programme 9"() -> (w292:cluster{"chaîne":string, "Valeur":dbl}[][])
              }
              frame "Prog 10" {
                n244 = local read "Programme 10"() -> (w294:cluster{"chaîne":string, "Valeur":dbl}[][])
              }
            }
            n245 = property on="Insérer segment" class="Bool"("Disabled"=w272) -> ()  [unwired: 2 in, 2 out]
            n246 = property on="Modif seg" class="Bool"("Disabled"=w272) -> ()  [unwired: 2 in, 2 out]
            n247 = property on="Ajouter segment" class="Bool"("Disabled"=w272) -> ()  [unwired: 2 in, 2 out]
            n248 = property on="Supprimer segment" class="Bool"("Disabled"=w272) -> ()  [unwired: 2 in, 2 out]
            n249 = property on="Sauvegarder" class="Bool"("Disabled"=w272) -> ()  [unwired: 2 in, 2 out]
            n250 = property on="Visualiser le profil" class="Bool"("Disabled"=w272) -> ()  [unwired: 2 in, 2 out]
            n251 = property on="Segment à éditer/supprimer" class="NumNb (strict)"("Disabled"=w272) -> ()  [unwired: 2 in, 2 out]
            n252 = property on="Onglet_segments" class="Onglet (strict)"("Disabled"=w272) -> ()  [unwired: 2 in, 2 out]
            n253 = call "Dernier_element_2D.vi"("Programme"=w271) -> ("Taille/Indice N+1"=w274:i32)  [unwired: 2 out]
            n254 = Equal To 0?(x=w274) -> (x = 0?=w273:bool)
            n255 = case shown="Vrai" w273 {
              tunnel: w271 -> [_ w305]
              tunnel: w270 -> [_ w299]
              tunnel: w269 -> [_ w296]
              frame False {
                n256 = One Button Dialog(message="Données générales déjà ajoutées.") -> ()  [unwired: 1 in, 1 out]
              }
              frame True {
                n257 = local read "Comm_Unité de rampe"() -> (w306:u16)
                n258 = local read "Comm_Unité de palier"() -> (w307:u16)
                n259 = local read "Configuration"() -> (w300:cluster{"Command (PV)":string, dbl}[])
                n260 = call "Generer_listing_alarmes.vi"("Configuration"=w300) -> ("Listing alarmes"=w301:string)
                n261 = call "Ajout_edition_segment EPC3000.vi"("Action"=enum16{"Edition", "Insertion", "Ajout"}."Ajout", "Numéro du segment"=u8 0 ("Numéro du segment à éditer"), "Programme_entrée"=w305, "Valeur 2"=u8 1, "Valeur 1"=w307, "Type de segment/Valeur 0"=w306) -> ("Programme_sortie"=w298:cluster{"chaîne":string, "Valeur":dbl}[][])  [unwired: 5 in]
                n262 = call "Generer_listing.vi"("Listing_entrée"=w301, "Numéro de programme"=w299, "Programme"=w298) -> ("Listing_sortie"=w297:string)
                n263 = case shown="\"Prog 10\"" w296 {
                  tunnel: w298 -> [w309 w311 w312 w315 w317 w318 w320 w323 w325 w327]
                  tunnel: w297 -> [w308 w310 w313 w314 w316 w319 w321 w322 w324 w326]
                  frame "Prog 1", Default {
                    n264 = local write "Listing programme 1"(w308) -> ()
                    n265 = local write "Programme 1"(w309) -> ()
                  }
                  frame "Prog 2" {
                    n266 = local write "Listing programme 2"(w310) -> ()
                    n267 = local write "Programme 2"(w311) -> ()
                  }
                  frame "Prog 3" {
                    n268 = local write "Listing programme 3"(w313) -> ()
                    n269 = local write "Programme 3"(w312) -> ()
                  }
                  frame "Prog 4" {
                    n270 = local write "Listing programme 4"(w314) -> ()
                    n271 = local write "Programme 4"(w315) -> ()
                  }
                  frame "Prog 5" {
                    n272 = local write "Listing programme 5"(w316) -> ()
                    n273 = local write "Programme 5"(w317) -> ()
                  }
                  frame "Prog 6" {
                    n274 = local write "Listing programme 6"(w319) -> ()
                    n275 = local write "Programme 6"(w318) -> ()
                  }
                  frame "Prog 7" {
                    n276 = local write "Listing programme 7"(w321) -> ()
                    n277 = local write "Programme 7"(w320) -> ()
                  }
                  frame "Prog 8" {
                    n278 = local write "Listing programme 8"(w322) -> ()
                    n279 = local write "Programme 8"(w323) -> ()
                  }
                  frame "Prog 9" {
                    n280 = local write "Listing programme 9"(w324) -> ()
                    n281 = local write "Programme 9"(w325) -> ()
                  }
                  frame "Prog 10" {
                    n282 = local write "Listing programme 10"(w326) -> ()
                    n283 = local write "Programme 10"(w327) -> ()
                  }
                }
              }
            }
          }
          event "Ajouter segment": Value Change {
            w339 = 1 ("y")
            # "Si dernier segment pas une fin de programme\nEt\nSi nombre de segments <26 (+données générales = 27)"
            n284 = event-data() -> ()  [unwired: 1 in, 6 out]
            n285 = property on="Onglets_programmes" class="Onglet (strict)"() -> ("Value"=w328:T1)  [unwired: 2 in, 2 out]
            n286 = case shown="\"Prog 10\"" w328 {
              tunnel: [w458 w460 w462 w464 w466 w468 w470 w472 w474 w476] -> w330
              tunnel: [u8 1 ("Numéro de programme") u8 2 ("Numéro de programme") u8 3 ("Numéro de programme") u8 4 ("Numéro de programme") u8 5 ("Numéro de programme") u8 6 ("Numéro de programme") u8 7 ("Numéro de programme") u8 8 ("Numéro de programme") u8 9 ("Numéro de programme") u8 10 ("Numéro de programme")] -> w329
              frame "Prog 1", Default {
                n287 = local read "Programme 1"() -> (w458:cluster{"chaîne":string, "Valeur":dbl}[][])
              }
              frame "Prog 2" {
                n288 = local read "Programme 2"() -> (w460:cluster{"chaîne":string, "Valeur":dbl}[][])
              }
              frame "Prog 3" {
                n289 = local read "Programme 3"() -> (w462:cluster{"chaîne":string, "Valeur":dbl}[][])
              }
              frame "Prog 4" {
                n290 = local read "Programme 4"() -> (w464:cluster{"chaîne":string, "Valeur":dbl}[][])
              }
              frame "Prog 5" {
                n291 = local read "Programme 5"() -> (w466:cluster{"chaîne":string, "Valeur":dbl}[][])
              }
              frame "Prog 6" {
                n292 = local read "Programme 6"() -> (w468:cluster{"chaîne":string, "Valeur":dbl}[][])
              }
              frame "Prog 7" {
                n293 = local read "Programme 7"() -> (w470:cluster{"chaîne":string, "Valeur":dbl}[][])
              }
              frame "Prog 8" {
                n294 = local read "Programme 8"() -> (w472:cluster{"chaîne":string, "Valeur":dbl}[][])
              }
              frame "Prog 9" {
                n295 = local read "Programme 9"() -> (w474:cluster{"chaîne":string, "Valeur":dbl}[][])
              }
              frame "Prog 10" {
                n296 = local read "Programme 10"() -> (w476:cluster{"chaîne":string, "Valeur":dbl}[][])
              }
            }
            n297 = call "Dernier_element_2D.vi"("Programme"=w330) -> ("Dernier segment"=w332:cluster{"chaîne":string, "Valeur":dbl}[], "Taille/Indice N+1"=w340:i32)  [unwired: 1 out]
            n298 = Index Array(array=w332, index=0 ("indice")) -> (element=w334:cluster{"chaîne":string, "Valeur":dbl})
            n299 = Unbundle(w334) -> ("Valeur"=w335:dbl)  [unwired: 1 out]
            n300 = Greater?(x=w340, y=w339) -> (0:w338:bool)
            n301 = Equal?(x=w340, y=w339) -> (x = y?=w341:bool)
            n302 = Equal To 0?(x=w335) -> (x = 0?=w337:bool)
            n303 = Less?(x=w340, y=27) -> (x < y?=w336:bool)
            n304 = And(x=w337, y=w341) -> (x .and. y?=w344:bool)
            n305 = Not And(1:w338, 2:w337) -> (0:w343:bool)
            n306 = Or(x=w344, y=w343) -> (x .or. y?=w342:bool)
            n307 = And(x=w342, y=w336) -> (x .and. y?=w331:bool)
            n308 = case shown="Vrai" w331 {
              tunnel: w330 -> [_ w354]
              tunnel: w329 -> [_ w350]
              tunnel: w328 -> [_ w349]
              frame False {
                n309 = One Button Dialog(message="Impossible d'ajouter un segment : \n- Soit le programme contient déjà 26 segments (+ les données générales) \n-Soit le dernier segment est une fin de programme.") -> ()  [unwired: 1 in, 1 out]
              }
              frame True {
                n310 = property on="Onglet_segments" class="Onglet (strict)"() -> ("Value"=w355:T2)  [unwired: 2 in, 2 out]
                n311 = case shown="\"Rampe en temps\"" w355 {
                  selector: w355 -> [w378 w390 w402 w413 w432 w448]
                  tunnel: [w380 w389 w401 w412 w431 w447] -> w348
                  tunnel: w354 -> [w379 w388 w400 w411 w430 w446]
                  tunnel: enum16{"Edition", "Insertion", "Ajout"}."Ajout" ("Action") -> [w377 w387 w399 w410 w429 w445]
                  frame "Fin de programme", Default {
                    n312 = call "Ajout_edition_segment EPC3000.vi"("Action"=w377, "Programme_entrée"=w379, "Valeur 1"="Type de fin", "Type de segment/Valeur 0"=w378) -> ("Programme_sortie"=w380:cluster{"chaîne":string, "Valeur":dbl}[][])  [unwired: 7 in]
                  }
                  frame "Saut" {
                    n313 = local read "Alarme haute"() -> (w386:dbl)
                    n314 = local read "Alarme basse"() -> (w385:dbl)
                    n315 = Greater Or Equal?(x="Cible saut (°C)", y=w386) -> (x >= y?=w384:bool)
                    n316 = Less Or Equal?(x="Cible saut (°C)", y=w385) -> (x <= y?=w383:bool)
                    n317 = Or(x=w384, y=w383) -> (x .or. y?=w382:bool)
                    n318 = case shown="Faux" w382 {
                      tunnel: w390 -> [w395 _]
                      tunnel: [w394 w397] -> w389
                      tunnel: w388 -> [w393 w397]
                      tunnel: w387 -> [w392 _]
                      tunnel: "Cible saut (°C)" -> [w391 _]
                      frame False {
                        n319 = call "Ajout_edition_segment EPC3000.vi"("Action"=w392, "Programme_entrée"=w393, "Valeur 1"=w391, "Type de segment/Valeur 0"=w395) -> ("Programme_sortie"=w394:cluster{"chaîne":string, "Valeur":dbl}[][])  [unwired: 7 in]
                      }
                      frame True {
                        n320 = One Button Dialog(message="Consigne incompatible avec les valeurs d'alarme") -> ()  [unwired: 1 in, 1 out]
                      }
                    }
                  }
                  frame "Palier" {
                    n321 = call "Ajout_edition_segment EPC3000.vi"("Action"=w399, "Programme_entrée"=w400, "Valeur 1"="Durée palier", "Type de segment/Valeur 0"=w402) -> ("Programme_sortie"=w401:cluster{"chaîne":string, "Valeur":dbl}[][])  [unwired: 7 in]
                  }
                  frame "Rampe en vitesse" {
                    n322 = local read "Alarme basse"() -> (w408:dbl)
                    n323 = local read "Alarme haute"() -> (w409:dbl)
                    n324 = Greater Or Equal?(x="Cible rampe vitesse", y=w409) -> (x >= y?=w407:bool)
                    n325 = Less Or Equal?(x="Cible rampe vitesse", y=w408) -> (x <= y?=w406:bool)
                    n326 = Or(x=w407, y=w406) -> (x .or. y?=w405:bool)
                    n327 = case shown="Faux" w405 {
                      tunnel: w413 -> [w419 _]
                      tunnel: [w418 w421] -> w412
                      tunnel: w411 -> [w417 w421]
                      tunnel: "Pente rampe vitesse" -> [w416 _]
                      tunnel: w410 -> [w415 _]
                      tunnel: "Cible rampe vitesse" -> [w414 _]
                      frame False {
                        n328 = call "Ajout_edition_segment EPC3000.vi"("Action"=w415, "Programme_entrée"=w417, "Valeur 2"=w416, "Valeur 1"=w414, "Type de segment/Valeur 0"=w419) -> ("Programme_sortie"=w418:cluster{"chaîne":string, "Valeur":dbl}[][])  [unwired: 6 in]
                      }
                      frame True {
                        n329 = One Button Dialog(message="Consigne incompatible avec les valeurs d'alarme") -> ()  [unwired: 1 in, 1 out]
                      }
                    }
                  }
                  frame "Rampe en temps" {
                    n330 = local read "Alarme basse"() -> (w427:dbl)
                    n331 = local read "Alarme haute"() -> (w428:dbl)
                    n332 = Greater Or Equal?(x="Cible rampe temps", y=w428) -> (x >= y?=w425:bool)
                    n333 = Less Or Equal?(x="Cible rampe temps", y=w427) -> (x <= y?=w426:bool)
                    n334 = Or(x=w425, y=w426) -> (x .or. y?=w424:bool)
                    n335 = case shown="Faux" w424 {
                      tunnel: w432 -> [w438 _]
                      tunnel: [w437 w440] -> w431
                      tunnel: w430 -> [w436 w440]
                      tunnel: "Durée rampe temps" -> [w435 _]
                      tunnel: w429 -> [w434 _]
                      tunnel: "Cible rampe temps" -> [w433 _]
                      frame False {
                        n336 = call "Ajout_edition_segment EPC3000.vi"("Action"=w434, "Programme_entrée"=w436, "Valeur 2"=w435, "Valeur 1"=w433, "Type de segment/Valeur 0"=w438) -> ("Programme_sortie"=w437:cluster{"chaîne":string, "Valeur":dbl}[][])  [unwired: 6 in]
                      }
                      frame True {
                        n337 = One Button Dialog(message="Consigne incompatible avec les valeurs d'alarme") -> ()  [unwired: 1 in, 1 out]
                      }
                    }
                  }
                  frame "Appel sous-programme" {
                    n338 = Equal?(x=u8 1 ("y"), y="Numéro prog") -> (x = y?=w444:bool)
                    n339 = case shown="Faux" w444 {
                      tunnel: w448 -> [w454 _]
                      tunnel: [w453 w456] -> w447
                      tunnel: w446 -> [w452 w456]
                      tunnel: "Nb cycles" -> [w451 _]
                      tunnel: w445 -> [w450 _]
                      tunnel: "Numéro prog" -> [w449 _]
                      frame False {
                        n340 = call "Ajout_edition_segment EPC3000.vi"("Action"=w450, "Programme_entrée"=w452, "Valeur 2"=w451, "Valeur 1"=w449, "Type de segment/Valeur 0"=w454) -> ("Programme_sortie"=w453:cluster{"chaîne":string, "Valeur":dbl}[][])  [unwired: 6 in]
                      }
                      frame True {
                        n341 = One Button Dialog(message="Il n'est pas possible d'appeler un numéro de sous programme identique au programme appelant ") -> ()  [unwired: 1 in, 1 out]
                      }
                    }
                  }
                }
                n342 = local read "Configuration"() -> (w351:cluster{"Command (PV)":string, dbl}[])
                n343 = call "Generer_listing_alarmes.vi"("Configuration"=w351) -> ("Listing alarmes"=w352:string)
                n344 = call "Generer_listing.vi"("Listing_entrée"=w352, "Numéro de programme"=w350, "Programme"=w348) -> ("Listing_sortie"=w347:string)
                n345 = case shown="\"Prog 10\"" w349 {
                  tunnel: w348 -> [w357 w359 w360 w363 w365 w366 w368 w371 w373 w375]
                  tunnel: w347 -> [w356 w358 w361 w362 w364 w367 w369 w370 w372 w374]
                  frame "Prog 1", Default {
                    n346 = local write "Listing programme 1"(w356) -> ()
                    n347 = local write "Programme 1"(w357) -> ()
                  }
                  frame "Prog 2" {
                    n348 = local write "Listing programme 2"(w358) -> ()
                    n349 = local write "Programme 2"(w359) -> ()
                  }
                  frame "Prog 3" {
                    n350 = local write "Listing programme 3"(w361) -> ()
                    n351 = local write "Programme 3"(w360) -> ()
                  }
                  frame "Prog 4" {
                    n352 = local write "Listing programme 4"(w362) -> ()
                    n353 = local write "Programme 4"(w363) -> ()
                  }
                  frame "Prog 5" {
                    n354 = local write "Listing programme 5"(w364) -> ()
                    n355 = local write "Programme 5"(w365) -> ()
                  }
                  frame "Prog 6" {
                    n356 = local write "Listing programme 6"(w367) -> ()
                    n357 = local write "Programme 6"(w366) -> ()
                  }
                  frame "Prog 7" {
                    n358 = local write "Listing programme 7"(w369) -> ()
                    n359 = local write "Programme 7"(w368) -> ()
                  }
                  frame "Prog 8" {
                    n360 = local write "Listing programme 8"(w370) -> ()
                    n361 = local write "Programme 8"(w371) -> ()
                  }
                  frame "Prog 9" {
                    n362 = local write "Listing programme 9"(w372) -> ()
                    n363 = local write "Programme 9"(w373) -> ()
                  }
                  frame "Prog 10" {
                    n364 = local write "Listing programme 10"(w374) -> ()
                    n365 = local write "Programme 10"(w375) -> ()
                  }
                }
              }
            }
          }
          event "Segment à éditer/supprimer": Value Change {
            n366 = event-data() -> ("NewVal"=w479:u8)  [unwired: 1 in, 5 out]
            n367 = property on="Onglets_programmes" class="Onglet (strict)"() -> ("Value"=w478:T1)  [unwired: 2 in, 2 out]
            n368 = case shown="\"Prog 1\", Par défaut" w478 {
              tunnel: [w491 w493 w495 w497 w499 w501 w503 w505 w507 w509] -> w477
              tunnel: [u8 1 ("Numéro de programme") u8 2 ("Numéro de programme") u8 3 ("Numéro de programme") u8 4 ("Numéro de programme") u8 5 ("Numéro de programme") u8 6 ("Numéro de programme") u8 7 ("Numéro de programme") u8 8 ("Numéro de programme") u8 9 ("Numéro de programme") u8 10 ("Numéro de programme")] -> _
              frame "Prog 1", Default {
                n369 = local read "Programme 1"() -> (w491:cluster{"chaîne":string, "Valeur":dbl}[][])
              }
              frame "Prog 2" {
                n370 = local read "Programme 2"() -> (w493:cluster{"chaîne":string, "Valeur":dbl}[][])
              }
              frame "Prog 3" {
                n371 = local read "Programme 3"() -> (w495:cluster{"chaîne":string, "Valeur":dbl}[][])
              }
              frame "Prog 4" {
                n372 = local read "Programme 4"() -> (w497:cluster{"chaîne":string, "Valeur":dbl}[][])
              }
              frame "Prog 5" {
                n373 = local read "Programme 5"() -> (w499:cluster{"chaîne":string, "Valeur":dbl}[][])
              }
              frame "Prog 6" {
                n374 = local read "Programme 6"() -> (w501:cluster{"chaîne":string, "Valeur":dbl}[][])
              }
              frame "Prog 7" {
                n375 = local read "Programme 7"() -> (w503:cluster{"chaîne":string, "Valeur":dbl}[][])
              }
              frame "Prog 8" {
                n376 = local read "Programme 8"() -> (w505:cluster{"chaîne":string, "Valeur":dbl}[][])
              }
              frame "Prog 9" {
                n377 = local read "Programme 9"() -> (w507:cluster{"chaîne":string, "Valeur":dbl}[][])
              }
              frame "Prog 10" {
                n378 = local read "Programme 10"() -> (w509:cluster{"chaîne":string, "Valeur":dbl}[][])
              }
            }
            n379 = case shown="Par défaut" w479 {
              selector: w479 -> [_ w486]
              tunnel: w477 -> [_ w485]
              frame 0 {
                # "Segment\ndonnées"
                n380 = for {
                  N: 10 -> [_]
                  shift-right: [w483] -> _
                  shift-left: TRUE -> [w482]
                  n381 = Wait (ms)(milliseconds to wait=u32 50 ("attente (ms)")) -> ()  [unwired: 1 out]
                  n382 = Not(x=w482) -> (.not. x?=w483:bool)
                  "Indicateur_Données à éditer" <- w482
                }
              }
              frame Default {
                # "Segment classique"
                # "Type de segment"
                n383 = Index Array(array=w485, index (row)=w486, index (col)=0 ("indice désactivé (col)")) -> (element=w488:cluster{"chaîne":string, "Valeur":dbl})
                n384 = Unbundle(w488) -> ("Valeur"=w487:dbl)  [unwired: 1 out]
                n385 = local write "Onglet_segments"(w487) -> ()
              }
            }
          }
          event "Modif seg": Value Change {
            n386 = event-data() -> ()  [unwired: 1 in, 6 out]
            n387 = local read "Segment à éditer/supprimer"() -> (w515:u8)
            n388 = Number To Decimal String(number=w515) -> (decimal integer string=w513:string)  [unwired: 1 in]
            n389 = Concatenate Strings("Confirmer l'édition du segment n°" ("message"), w513, "?" ("chaîne")) -> (w511:string)
            n390 = Two Button Dialog(message=w511) -> (T button?=w510:bool)  [unwired: 2 in]
            n391 = case shown="Vrai" w510 {
              frame False {
              }
              frame True {
                n392 = property on="Onglets_programmes" class="Onglet (strict)"() -> ("Value"=w516:T1)  [unwired: 2 in, 2 out]
                n393 = case shown="\"Prog 10\"" w516 {
                  tunnel: [w524 w526 w528 w530 w532 w534 w536 w538 w540 w542] -> w518
                  tunnel: [u8 1 ("Numéro de programme") u8 2 ("Numéro de programme") u8 3 ("Numéro de programme") u8 4 ("Numéro de programme") u8 5 ("Numéro de programme") u8 6 ("Numéro de programme") u8 7 ("Numéro de programme") u8 8 ("Numéro de programme") u8 9 ("Numéro de programme") u8 10 ("Numéro de programme")] -> w517
                  frame "Prog 1", Default {
                    n394 = local read "Programme 1"() -> (w524:cluster{"chaîne":string, "Valeur":dbl}[][])
                  }
                  frame "Prog 2" {
                    n395 = local read "Programme 2"() -> (w526:cluster{"chaîne":string, "Valeur":dbl}[][])
                  }
                  frame "Prog 3" {
                    n396 = local read "Programme 3"() -> (w528:cluster{"chaîne":string, "Valeur":dbl}[][])
                  }
                  frame "Prog 4" {
                    n397 = local read "Programme 4"() -> (w530:cluster{"chaîne":string, "Valeur":dbl}[][])
                  }
                  frame "Prog 5" {
                    n398 = local read "Programme 5"() -> (w532:cluster{"chaîne":string, "Valeur":dbl}[][])
                  }
                  frame "Prog 6" {
                    n399 = local read "Programme 6"() -> (w534:cluster{"chaîne":string, "Valeur":dbl}[][])
                  }
                  frame "Prog 7" {
                    n400 = local read "Programme 7"() -> (w536:cluster{"chaîne":string, "Valeur":dbl}[][])
                  }
                  frame "Prog 8" {
                    n401 = local read "Programme 8"() -> (w538:cluster{"chaîne":string, "Valeur":dbl}[][])
                  }
                  frame "Prog 9" {
                    n402 = local read "Programme 9"() -> (w540:cluster{"chaîne":string, "Valeur":dbl}[][])
                  }
                  frame "Prog 10" {
                    n403 = local read "Programme 10"() -> (w542:cluster{"chaîne":string, "Valeur":dbl}[][])
                  }
                }
                n404 = local read "Segment à éditer/supprimer"() -> (w520:u8)
                n405 = call "Dernier_element_2D.vi"("Programme"=w518) -> ("Indice N"=w519:i32)  [unwired: 2 out]
                n406 = Less Or Equal?(x=w520, y=w519) -> (x <= y?=w521:bool)
                n407 = case shown="Vrai" w521 {
                  tunnel: w520 -> [_ w552]
                  tunnel: w518 -> [_ w551]
                  tunnel: enum16{"Edition", "Insertion", "Ajout"}."Edition" ("Action") -> [_ w550]
                  tunnel: w517 -> [_ w545]
                  tunnel: w516 -> [_ w544]
                  frame False {
                    n408 = One Button Dialog(message="Impossible d'éditer un segment inexistant !") -> ()  [unwired: 1 in, 1 out]
                  }
                  frame True {
                    n409 = case shown="0" w552 {
                      selector: w552 -> [w576 w675]
                      tunnel: w551 -> [w574 w673]
                      tunnel: [w573 w674] -> w547
                      tunnel: w550 -> [w575 w669]
                      frame Default {
                        # "Segment classique"
                        n410 = property on="Onglet_segments" class="Onglet (strict)"() -> ("Value"=w577:T2)  [unwired: 2 in, 2 out]
                        n411 = case shown="\"Saut\"" w577 {
                          selector: w577 -> [w580 w594 w608 w620 w641 w659]
                          tunnel: [w582 w593 w606 w619 w640 w658] -> w573
                          tunnel: w574 -> [w581 w592 w605 w618 w639 w657]
                          tunnel: w575 -> [w579 w591 w604 w616 w637 w655]
                          tunnel: w576 -> [w578 w584 w603 w609 w630 w651]
                          frame "Fin de programme", Default {
                            n412 = local read "Type de fin"() -> (w583:u8)
                            n413 = call "Ajout_edition_segment EPC3000.vi"("Action"=w579, "Numéro du segment"=w578, "Programme_entrée"=w581, "Valeur 1"=w583, "Type de segment/Valeur 0"=w580) -> ("Programme_sortie"=w582:cluster{"chaîne":string, "Valeur":dbl}[][])  [unwired: 6 in]
                          }
                          frame "Saut" {
                            n414 = local read "Cible saut (°C)"() -> (w589:dbl)
                            n415 = local read "Alarme haute"() -> (w590:dbl)
                            n416 = local read "Alarme basse"() -> (w588:dbl)
                            n417 = Greater Or Equal?(x=w589, y=w590) -> (x >= y?=w587:bool)
                            n418 = Less Or Equal?(x=w589, y=w588) -> (x <= y?=w586:bool)
                            n419 = Or(x=w587, y=w586) -> (x .or. y?=w585:bool)
                            n420 = case shown="Faux" w585 {
                              tunnel: w594 -> [w600 _]
                              tunnel: [w599 w602] -> w593
                              tunnel: w592 -> [w598 w602]
                              tunnel: w591 -> [w597 _]
                              tunnel: w589 -> [w596 _]
                              tunnel: w584 -> [w595 _]
                              frame False {
                                n421 = call "Ajout_edition_segment EPC3000.vi"("Action"=w597, "Numéro du segment"=w595, "Programme_entrée"=w598, "Valeur 1"=w596, "Type de segment/Valeur 0"=w600) -> ("Programme_sortie"=w599:cluster{"chaîne":string, "Valeur":dbl}[][])  [unwired: 6 in]
                              }
                              frame True {
                                n422 = One Button Dialog(message="Consigne incompatible avec les valeurs d'alarme") -> ()  [unwired: 1 in, 1 out]
                              }
                            }
                          }
                          frame "Palier" {
                            n423 = local read "Durée palier"() -> (w607:sgl)
                            n424 = call "Ajout_edition_segment EPC3000.vi"("Action"=w604, "Numéro du segment"=w603, "Programme_entrée"=w605, "Valeur 1"=w607, "Type de segment/Valeur 0"=w608) -> ("Programme_sortie"=w606:cluster{"chaîne":string, "Valeur":dbl}[][])  [unwired: 6 in]
                          }
                          frame "Rampe en vitesse" {
                            n425 = local read "Cible rampe vitesse"() -> (w614:dbl)
                            n426 = local read "Alarme haute"() -> (w615:dbl)
                            n427 = local read "Alarme basse"() -> (w613:dbl)
                            n428 = local read "Pente rampe vitesse"() -> (w617:sgl)
                            n429 = Greater Or Equal?(x=w614, y=w615) -> (x >= y?=w612:bool)
                            n430 = Less Or Equal?(x=w614, y=w613) -> (x <= y?=w611:bool)
                            n431 = Or(x=w612, y=w611) -> (x .or. y?=w610:bool)
                            n432 = case shown="Faux" w610 {
                              tunnel: w620 -> [w627 _]
                              tunnel: [w626 w629] -> w619
                              tunnel: w618 -> [w625 w629]
                              tunnel: w617 -> [w624 _]
                              tunnel: w616 -> [w623 _]
                              tunnel: w614 -> [w622 _]
                              tunnel: w609 -> [w621 _]
                              frame False {
                                n433 = call "Ajout_edition_segment EPC3000.vi"("Action"=w623, "Numéro du segment"=w621, "Programme_entrée"=w625, "Valeur 2"=w624, "Valeur 1"=w622, "Type de segment/Valeur 0"=w627) -> ("Programme_sortie"=w626:cluster{"chaîne":string, "Valeur":dbl}[][])  [unwired: 5 in]
                              }
                              frame True {
                                n434 = One Button Dialog(message="Consigne incompatible avec les valeurs d'alarme") -> ()  [unwired: 1 in, 1 out]
                              }
                            }
                          }
                          frame "Rampe en temps" {
                            n435 = local read "Cible rampe temps"() -> (w635:dbl)
                            n436 = local read "Alarme basse"() -> (w634:dbl)
                            n437 = local read "Alarme haute"() -> (w636:dbl)
                            n438 = local read "Durée rampe temps"() -> (w638:sgl)
                            n439 = Greater Or Equal?(x=w635, y=w636) -> (x >= y?=w632:bool)
                            n440 = Less Or Equal?(x=w635, y=w634) -> (x <= y?=w633:bool)
                            n441 = Or(x=w632, y=w633) -> (x .or. y?=w631:bool)
                            n442 = case shown="Faux" w631 {
                              tunnel: w641 -> [w648 _]
                              tunnel: [w647 w650] -> w640
                              tunnel: w639 -> [w646 w650]
                              tunnel: w638 -> [w645 _]
                              tunnel: w637 -> [w644 _]
                              tunnel: w635 -> [w643 _]
                              tunnel: w630 -> [w642 _]
                              frame False {
                                n443 = call "Ajout_edition_segment EPC3000.vi"("Action"=w644, "Numéro du segment"=w642, "Programme_entrée"=w646, "Valeur 2"=w645, "Valeur 1"=w643, "Type de segment/Valeur 0"=w648) -> ("Programme_sortie"=w647:cluster{"chaîne":string, "Valeur":dbl}[][])  [unwired: 5 in]
                              }
                              frame True {
                                n444 = One Button Dialog(message="Consigne incompatible avec les valeurs d'alarme") -> ()  [unwired: 1 in, 1 out]
                              }
                            }
                          }
                          frame "Appel sous-programme" {
                            n445 = local read "Numéro prog"() -> (w652:u8)
                            n446 = local read "Nb cycles"() -> (w656:u8)
                            n447 = Equal?(x=u8 1 ("y"), y=w652) -> (x = y?=w654:bool)
                            n448 = case shown="Faux" w654 {
                              tunnel: w659 -> [w666 _]
                              tunnel: [w665 w668] -> w658
                              tunnel: w657 -> [w664 w668]
                              tunnel: w656 -> [w663 _]
                              tunnel: w655 -> [w662 _]
                              tunnel: w652 -> [w661 _]
                              tunnel: w651 -> [w660 _]
                              frame False {
                                n449 = call "Ajout_edition_segment EPC3000.vi"("Action"=w662, "Numéro du segment"=w660, "Programme_entrée"=w664, "Valeur 2"=w663, "Valeur 1"=w661, "Type de segment/Valeur 0"=w666) -> ("Programme_sortie"=w665:cluster{"chaîne":string, "Valeur":dbl}[][])  [unwired: 5 in]
                              }
                              frame True {
                                n450 = One Button Dialog(message="Il n'est pas possible d'appeler un numéro de sous programme identique au programme appelant ") -> ()  [unwired: 1 in, 1 out]
                              }
                            }
                          }
                        }
                      }
                      frame 0 {
                        # "Données générales"
                        n451 = local read "Comm_Unité de palier"() -> (w671:u16)
                        n452 = local read "Comm_Unité de rampe"() -> (w672:u16)
                        n453 = call "Ajout_edition_segment EPC3000.vi"("Action"=w669, "Numéro du segment"=w675, "Programme_entrée"=w673, "Valeur 2"=u8 1, "Valeur 1"=w671, "Type de segment/Valeur 0"=w672) -> ("Programme_sortie"=w674:cluster{"chaîne":string, "Valeur":dbl}[][])  [unwired: 5 in]
                      }
                    }
                    n454 = local read "Configuration"() -> (w548:cluster{"Command (PV)":string, dbl}[])
                    n455 = call "Generer_listing_alarmes.vi"("Configuration"=w548) -> ("Listing alarmes"=w549:string)
                    n456 = call "Generer_listing.vi"("Listing_entrée"=w549, "Numéro de programme"=w545, "Programme"=w547) -> ("Listing_sortie"=w546:string)
                    n457 = case shown="\"Prog 10\"" w544 {
                      tunnel: w547 -> [w554 w556 w557 w560 w562 w563 w565 w568 w570 w572]
                      tunnel: w546 -> [w553 w555 w558 w559 w561 w564 w566 w567 w569 w571]
                      frame "Prog 1", Default {
                        n458 = local write "Listing programme 1"(w553) -> ()
                        n459 = local write "Programme 1"(w554) -> ()
                      }
                      frame "Prog 2" {
                        n460 = local write "Listing programme 2"(w555) -> ()
                        n461 = local write "Programme 2"(w556) -> ()
                      }
                      frame "Prog 3" {
                        n462 = local write "Listing programme 3"(w558) -> ()
                        n463 = local write "Programme 3"(w557) -> ()
                      }
                      frame "Prog 4" {
                        n464 = local write "Listing programme 4"(w559) -> ()
                        n465 = local write "Programme 4"(w560) -> ()
                      }
                      frame "Prog 5" {
                        n466 = local write "Listing programme 5"(w561) -> ()
                        n467 = local write "Programme 5"(w562) -> ()
                      }
                      frame "Prog 6" {
                        n468 = local write "Listing programme 6"(w564) -> ()
                        n469 = local write "Programme 6"(w563) -> ()
                      }
                      frame "Prog 7" {
                        n470 = local write "Listing programme 7"(w566) -> ()
                        n471 = local write "Programme 7"(w565) -> ()
                      }
                      frame "Prog 8" {
                        n472 = local write "Listing programme 8"(w567) -> ()
                        n473 = local write "Programme 8"(w568) -> ()
                      }
                      frame "Prog 9" {
                        n474 = local write "Listing programme 9"(w569) -> ()
                        n475 = local write "Programme 9"(w570) -> ()
                      }
                      frame "Prog 10" {
                        n476 = local write "Listing programme 10"(w571) -> ()
                        n477 = local write "Programme 10"(w572) -> ()
                      }
                    }
                  }
                }
              }
            }
          }
          event "Insérer segment": Value Change {
            n478 = event-data() -> ()  [unwired: 1 in, 2 out]
            n479 = local read "Segment à éditer/supprimer"() -> (w677:u8)
            n480 = Equal To 0?(x=w677) -> (x = 0?=w676:bool)
            n481 = case shown="Faux" w676 {
              tunnel: w677 -> [_ w679]
              frame True {
                n482 = One Button Dialog(message="Impossible d'insérer un segment à l'indice 0.") -> ()  [unwired: 1 in, 1 out]
              }
              frame False {
                n483 = Number To Decimal String(number=w679) -> (decimal integer string=w683:string)  [unwired: 1 in]
                n484 = Concatenate Strings("Confirmer l'insertion du segment à l'indice n°" ("message"), w683, "?" ("chaîne")) -> (w681:string)
                n485 = Two Button Dialog(message=w681) -> (T button?=w680:bool)  [unwired: 2 in]
                n486 = case shown="Vrai" w680 {
                  frame False {
                  }
                  frame True {
                    n487 = property on="Onglets_programmes" class="Onglet (strict)"() -> ("Value"=w685:T1)  [unwired: 2 in, 2 out]
                    n488 = case shown="\"Prog 10\"" w685 {
                      tunnel: [w825 w827 w829 w831 w833 w835 w837 w839 w841 w843] -> w686
                      tunnel: [u8 1 ("Numéro de programme") u8 2 ("Numéro de programme") u8 3 ("Numéro de programme") u8 4 ("Numéro de programme") u8 5 ("Numéro de programme") u8 6 ("Numéro de programme") u8 7 ("Numéro de programme") u8 8 ("Numéro de programme") u8 9 ("Numéro de programme") u8 10 ("Numéro de programme")] -> w687
                      frame "Prog 1", Default {
                        n489 = local read "Programme 1"() -> (w825:cluster{"chaîne":string, "Valeur":dbl}[][])
                      }
                      frame "Prog 2" {
                        n490 = local read "Programme 2"() -> (w827:cluster{"chaîne":string, "Valeur":dbl}[][])
                      }
                      frame "Prog 3" {
                        n491 = local read "Programme 3"() -> (w829:cluster{"chaîne":string, "Valeur":dbl}[][])
                      }
                      frame "Prog 4" {
                        n492 = local read "Programme 4"() -> (w831:cluster{"chaîne":string, "Valeur":dbl}[][])
                      }
                      frame "Prog 5" {
                        n493 = local read "Programme 5"() -> (w833:cluster{"chaîne":string, "Valeur":dbl}[][])
                      }
                      frame "Prog 6" {
                        n494 = local read "Programme 6"() -> (w835:cluster{"chaîne":string, "Valeur":dbl}[][])
                      }
                      frame "Prog 7" {
                        n495 = local read "Programme 7"() -> (w837:cluster{"chaîne":string, "Valeur":dbl}[][])
                      }
                      frame "Prog 8" {
                        n496 = local read "Programme 8"() -> (w839:cluster{"chaîne":string, "Valeur":dbl}[][])
                      }
                      frame "Prog 9" {
                        n497 = local read "Programme 9"() -> (w841:cluster{"chaîne":string, "Valeur":dbl}[][])
                      }
                      frame "Prog 10" {
                        n498 = local read "Programme 10"() -> (w843:cluster{"chaîne":string, "Valeur":dbl}[][])
                      }
                    }
                    n499 = call "Dernier_element_2D.vi"("Programme"=w686) -> ("Taille/Indice N+1"=w690:i32)  [unwired: 2 out]
                    n500 = Less?(x=w690, y=27 ("cas vrai")) -> (x < y?=w689:bool)
                    n501 = case shown="Vrai" w689 {
                      tunnel: w686 -> [_ w698]
                      tunnel: w687 -> [_ w695]
                      tunnel: w685 -> [_ w692]
                      frame False {
                        n502 = One Button Dialog(message="Trop de segments - Insertion impossible") -> ()  [unwired: 1 in, 1 out]
                      }
                      frame True {
                        n503 = local read "Segment à éditer/supprimer"() -> (w700:u8)
                        n504 = case shown="Par défaut" w700 {
                          selector: w700 -> [w723 w823]
                          tunnel: w698 -> [w722 w821]
                          tunnel: [w721 w822] -> w694
                          tunnel: enum16{"Edition", "Insertion", "Ajout"}."Insertion" ("Action") -> [w724 w817]
                          frame Default {
                            # "Segment classique"
                            n505 = property on="Onglet_segments" class="Onglet (strict)"() -> ("Value"=w725:T2)  [unwired: 2 in, 2 out]
                            n506 = case shown="\"Fin de programme\", Par défaut" w725 {
                              selector: w725 -> [w728 w742 w756 w768 w789 w807]
                              tunnel: [w730 w741 w754 w767 w788 w806] -> w721
                              tunnel: w722 -> [w729 w740 w753 w766 w787 w805]
                              tunnel: w724 -> [w727 w739 w752 w764 w785 w803]
                              tunnel: w723 -> [w726 w732 w751 w757 w778 w799]
                              frame "Fin de programme", Default {
                                n507 = local read "Type de fin"() -> (w731:u8)
                                n508 = call "Ajout_edition_segment EPC3000.vi"("Action"=w727, "Numéro du segment"=w726, "Programme_entrée"=w729, "Valeur 1"=w731, "Type de segment/Valeur 0"=w728) -> ("Programme_sortie"=w730:cluster{"chaîne":string, "Valeur":dbl}[][])  [unwired: 6 in]
                              }
                              frame "Saut" {
                                n509 = local read "Cible saut (°C)"() -> (w737:dbl)
                                n510 = local read "Alarme haute"() -> (w738:dbl)
                                n511 = local read "Alarme basse"() -> (w736:dbl)
                                n512 = Greater Or Equal?(x=w737, y=w738) -> (x >= y?=w735:bool)
                                n513 = Less Or Equal?(x=w737, y=w736) -> (x <= y?=w734:bool)
                                n514 = Or(x=w735, y=w734) -> (x .or. y?=w733:bool)
                                n515 = case shown="Faux" w733 {
                                tunnel: w742 -> [w748 _]
                                tunnel: [w747 w750] -> w741
                                tunnel: w740 -> [w746 w750]
                                tunnel: w739 -> [w745 _]
                                tunnel: w737 -> [w744 _]
                                tunnel: w732 -> [w743 _]
                                frame False {
                                n516 = call "Ajout_edition_segment EPC3000.vi"("Action"=w745, "Numéro du segment"=w743, "Programme_entrée"=w746, "Valeur 1"=w744, "Type de segment/Valeur 0"=w748) -> ("Programme_sortie"=w747:cluster{"chaîne":string, "Valeur":dbl}[][])  [unwired: 6 in]
                                }
                                frame True {
                                n517 = One Button Dialog(message="Consigne incompatible avec les valeurs d'alarme") -> ()  [unwired: 1 in, 1 out]
                                }
                                }
                              }
                              frame "Palier" {
                                n518 = local read "Durée palier"() -> (w755:sgl)
                                n519 = call "Ajout_edition_segment EPC3000.vi"("Action"=w752, "Numéro du segment"=w751, "Programme_entrée"=w753, "Valeur 1"=w755, "Type de segment/Valeur 0"=w756) -> ("Programme_sortie"=w754:cluster{"chaîne":string, "Valeur":dbl}[][])  [unwired: 6 in]
                              }
                              frame "Rampe en vitesse" {
                                n520 = local read "Cible rampe vitesse"() -> (w762:dbl)
                                n521 = local read "Alarme basse"() -> (w761:dbl)
                                n522 = local read "Alarme haute"() -> (w763:dbl)
                                n523 = local read "Pente rampe vitesse"() -> (w765:sgl)
                                n524 = Greater Or Equal?(x=w762, y=w763) -> (x >= y?=w760:bool)
                                n525 = Less Or Equal?(x=w762, y=w761) -> (x <= y?=w759:bool)
                                n526 = Or(x=w760, y=w759) -> (x .or. y?=w758:bool)
                                n527 = case shown="Faux" w758 {
                                tunnel: w768 -> [w775 _]
                                tunnel: [w774 w777] -> w767
                                tunnel: w766 -> [w773 w777]
                                tunnel: w765 -> [w772 _]
                                tunnel: w764 -> [w771 _]
                                tunnel: w762 -> [w770 _]
                                tunnel: w757 -> [w769 _]
                                frame False {
                                n528 = call "Ajout_edition_segment EPC3000.vi"("Action"=w771, "Numéro du segment"=w769, "Programme_entrée"=w773, "Valeur 2"=w772, "Valeur 1"=w770, "Type de segment/Valeur 0"=w775) -> ("Programme_sortie"=w774:cluster{"chaîne":string, "Valeur":dbl}[][])  [unwired: 5 in]
                                }
                                frame True {
                                n529 = One Button Dialog(message="Consigne incompatible avec les valeurs d'alarme") -> ()  [unwired: 1 in, 1 out]
                                }
                                }
                              }
                              frame "Rampe en temps" {
                                n530 = local read "Cible rampe temps"() -> (w783:dbl)
                                n531 = local read "Alarme haute"() -> (w784:dbl)
                                n532 = local read "Alarme basse"() -> (w782:dbl)
                                n533 = local read "Durée rampe temps"() -> (w786:sgl)
                                n534 = Greater Or Equal?(x=w783, y=w784) -> (x >= y?=w780:bool)
                                n535 = Less Or Equal?(x=w783, y=w782) -> (x <= y?=w781:bool)
                                n536 = Or(x=w780, y=w781) -> (x .or. y?=w779:bool)
                                n537 = case shown="Faux" w779 {
                                tunnel: w789 -> [w796 _]
                                tunnel: [w795 w798] -> w788
                                tunnel: w787 -> [w794 w798]
                                tunnel: w786 -> [w793 _]
                                tunnel: w785 -> [w792 _]
                                tunnel: w783 -> [w791 _]
                                tunnel: w778 -> [w790 _]
                                frame False {
                                n538 = call "Ajout_edition_segment EPC3000.vi"("Action"=w792, "Numéro du segment"=w790, "Programme_entrée"=w794, "Valeur 2"=w793, "Valeur 1"=w791, "Type de segment/Valeur 0"=w796) -> ("Programme_sortie"=w795:cluster{"chaîne":string, "Valeur":dbl}[][])  [unwired: 5 in]
                                }
                                frame True {
                                n539 = One Button Dialog(message="Consigne incompatible avec les valeurs d'alarme") -> ()  [unwired: 1 in, 1 out]
                                }
                                }
                              }
                              frame "Appel sous-programme" {
                                n540 = local read "Numéro prog"() -> (w800:u8)
                                n541 = local read "Nb cycles"() -> (w804:u8)
                                n542 = Equal?(x=u8 1 ("y"), y=w800) -> (x = y?=w802:bool)
                                n543 = case shown="Faux" w802 {
                                tunnel: w807 -> [w814 _]
                                tunnel: [w813 w816] -> w806
                                tunnel: w805 -> [w812 w816]
                                tunnel: w804 -> [w811 _]
                                tunnel: w803 -> [w810 _]
                                tunnel: w800 -> [w809 _]
                                tunnel: w799 -> [w808 _]
                                frame False {
                                n544 = call "Ajout_edition_segment EPC3000.vi"("Action"=w810, "Numéro du segment"=w808, "Programme_entrée"=w812, "Valeur 2"=w811, "Valeur 1"=w809, "Type de segment/Valeur 0"=w814) -> ("Programme_sortie"=w813:cluster{"chaîne":string, "Valeur":dbl}[][])  [unwired: 5 in]
                                }
                                frame True {
                                n545 = One Button Dialog(message="Il n'est pas possible d'appeler un numéro de sous programme identique au programme appelant ") -> ()  [unwired: 1 in, 1 out]
                                }
                                }
                              }
                            }
                          }
                          frame 0 {
                            # "Données générales"
                            n546 = local read "Comm_Unité de palier"() -> (w819:u16)
                            n547 = local read "Comm_Unité de rampe"() -> (w820:u16)
                            n548 = call "Ajout_edition_segment EPC3000.vi"("Action"=w817, "Numéro du segment"=w823, "Programme_entrée"=w821, "Valeur 2"=u8 1, "Valeur 1"=w819, "Type de segment/Valeur 0"=w820) -> ("Programme_sortie"=w822:cluster{"chaîne":string, "Valeur":dbl}[][])  [unwired: 5 in]
                          }
                        }
                        n549 = local read "Configuration"() -> (w696:cluster{"Command (PV)":string, dbl}[])
                        n550 = call "Generer_listing_alarmes.vi"("Configuration"=w696) -> ("Listing alarmes"=w697:string)
                        n551 = call "Generer_listing.vi"("Listing_entrée"=w697, "Numéro de programme"=w695, "Programme"=w694) -> ("Listing_sortie"=w693:string)
                        n552 = case shown="\"Prog 10\"" w692 {
                          tunnel: w694 -> [w702 w704 w705 w708 w710 w711 w713 w716 w718 w720]
                          tunnel: w693 -> [w701 w703 w706 w707 w709 w712 w714 w715 w717 w719]
                          frame "Prog 1", Default {
                            n553 = local write "Listing programme 1"(w701) -> ()
                            n554 = local write "Programme 1"(w702) -> ()
                          }
                          frame "Prog 2" {
                            n555 = local write "Listing programme 2"(w703) -> ()
                            n556 = local write "Programme 2"(w704) -> ()
                          }
                          frame "Prog 3" {
                            n557 = local write "Listing programme 3"(w706) -> ()
                            n558 = local write "Programme 3"(w705) -> ()
                          }
                          frame "Prog 4" {
                            n559 = local write "Listing programme 4"(w707) -> ()
                            n560 = local write "Programme 4"(w708) -> ()
                          }
                          frame "Prog 5" {
                            n561 = local write "Listing programme 5"(w709) -> ()
                            n562 = local write "Programme 5"(w710) -> ()
                          }
                          frame "Prog 6" {
                            n563 = local write "Listing programme 6"(w712) -> ()
                            n564 = local write "Programme 6"(w711) -> ()
                          }
                          frame "Prog 7" {
                            n565 = local write "Listing programme 7"(w714) -> ()
                            n566 = local write "Programme 7"(w713) -> ()
                          }
                          frame "Prog 8" {
                            n567 = local write "Listing programme 8"(w715) -> ()
                            n568 = local write "Programme 8"(w716) -> ()
                          }
                          frame "Prog 9" {
                            n569 = local write "Listing programme 9"(w717) -> ()
                            n570 = local write "Programme 9"(w718) -> ()
                          }
                          frame "Prog 10" {
                            n571 = local write "Listing programme 10"(w719) -> ()
                            n572 = local write "Programme 10"(w720) -> ()
                          }
                        }
                      }
                    }
                  }
                }
              }
            }
          }
          event "Supprimer segment": Value Change {
            n573 = event-data() -> ()  [unwired: 1 in, 6 out]
            n574 = local read "Segment à éditer/supprimer"() -> (w845:u8)
            n575 = Equal To 0?(x=w845) -> (x = 0?=w844:bool)
            n576 = case shown="Faux" w844 {
              frame True {
                n577 = One Button Dialog(message="Impossible de supprimer le segment 0.") -> ()  [unwired: 1 in, 1 out]
              }
              frame False {
                n578 = local read "Segment à éditer/supprimer"() -> (w852:u8)
                n579 = Number To Decimal String(number=w852) -> (decimal integer string=w850:string)  [unwired: 1 in]
                n580 = Concatenate Strings("Confirmer la suppression du segment n°" ("message"), w850, "?" ("chaîne")) -> (w848:string)
                n581 = Two Button Dialog(message=w848) -> (T button?=w847:bool)  [unwired: 2 in]
                n582 = case shown="Vrai" w847 {
                  frame False {
                  }
                  frame True {
                    # "Si données générales écrites\non a :\nTaille_programme >= 1"
                    n583 = property on="Onglets_programmes" class="Onglet (strict)"() -> ("Value"=w853:T1)  [unwired: 2 in, 2 out]
                    n584 = case shown="\"Prog 10\"" w853 {
                      tunnel: [w887 w889 w891 w893 w895 w897 w899 w901 w903 w905] -> w857
                      tunnel: [u8 1 ("Numéro de programme") u8 2 ("Numéro de programme") u8 3 ("Numéro de programme") u8 4 ("Numéro de programme") u8 5 ("Numéro de programme") u8 6 ("Numéro de programme") u8 7 ("Numéro de programme") u8 8 ("Numéro de programme") u8 9 ("Numéro de programme") u8 10 ("Numéro de programme")] -> w856
                      frame "Prog 1", Default {
                        n585 = local read "Programme 1"() -> (w887:cluster{"chaîne":string, "Valeur":dbl}[][])
                      }
                      frame "Prog 2" {
                        n586 = local read "Programme 2"() -> (w889:cluster{"chaîne":string, "Valeur":dbl}[][])
                      }
                      frame "Prog 3" {
                        n587 = local read "Programme 3"() -> (w891:cluster{"chaîne":string, "Valeur":dbl}[][])
                      }
                      frame "Prog 4" {
                        n588 = local read "Programme 4"() -> (w893:cluster{"chaîne":string, "Valeur":dbl}[][])
                      }
                      frame "Prog 5" {
                        n589 = local read "Programme 5"() -> (w895:cluster{"chaîne":string, "Valeur":dbl}[][])
                      }
                      frame "Prog 6" {
                        n590 = local read "Programme 6"() -> (w897:cluster{"chaîne":string, "Valeur":dbl}[][])
                      }
                      frame "Prog 7" {
                        n591 = local read "Programme 7"() -> (w899:cluster{"chaîne":string, "Valeur":dbl}[][])
                      }
                      frame "Prog 8" {
                        n592 = local read "Programme 8"() -> (w901:cluster{"chaîne":string, "Valeur":dbl}[][])
                      }
                      frame "Prog 9" {
                        n593 = local read "Programme 9"() -> (w903:cluster{"chaîne":string, "Valeur":dbl}[][])
                      }
                      frame "Prog 10" {
                        n594 = local read "Programme 10"() -> (w905:cluster{"chaîne":string, "Valeur":dbl}[][])
                      }
                    }
                    n595 = local read "Segment à éditer/supprimer"() -> (w863:u8)
                    n596 = call "Suppression_segment EPC.vi"("Programme_entrée"=w857, "Numéro du segment à supprimer"=w863) -> ("Programme_sortie"=w855:cluster{"chaîne":string, "Valeur":dbl}[][])
                    n597 = local read "Configuration"() -> (w859:cluster{"Command (PV)":string, dbl}[])
                    n598 = call "Dernier_element_2D.vi"("Programme"=w855) -> ("Taille/Indice N+1"=w858:i32)  [unwired: 2 out]
                    n599 = Greater Or Equal?(x=w858, y=1) -> (x >= y?=w862:bool)
                    n600 = case shown="Faux" w862 {
                      frame True {
                        w884 = u8 0 ("Désactivé")
                        # "Controles activés"
                        # "Données générales écrites"
                        n601 = property on="Modif seg" class="Bool"("Disabled"=w884) -> ()  [unwired: 2 in, 2 out]
                        n602 = property on="Ajouter segment" class="Bool"("Disabled"=w884) -> ()  [unwired: 2 in, 2 out]
                        n603 = property on="Onglet_segments" class="Onglet (strict)"("Disabled"=w884) -> ()  [unwired: 2 in, 2 out]
                        n604 = property on="Supprimer segment" class="Bool"("Disabled"=w884) -> ()  [unwired: 2 in, 2 out]
                        n605 = property on="Insérer segment" class="Bool"("Disabled"=w884) -> ()  [unwired: 2 in, 2 out]
                        n606 = property on="Sauvegarder" class="Bool"("Disabled"=w884) -> ()  [unwired: 2 in, 2 out]
                        n607 = property on="Visualiser le profil" class="Bool"("Disabled"=w884) -> ()  [unwired: 2 in, 2 out]
                        n608 = property on="Segment à éditer/supprimer" class="NumNb (strict)"("Disabled"=w884) -> ()  [unwired: 2 in, 2 out]
                      }
                      frame False {
                        w885 = u8 2 ("Désactivé")
                        # "Controles desactivés"
                        # "Données générales non écrites"
                        n609 = property on="Modif seg" class="Bool"("Disabled"=w885) -> ()  [unwired: 2 in, 2 out]
                        n610 = property on="Ajouter segment" class="Bool"("Disabled"=w885) -> ()  [unwired: 2 in, 2 out]
                        n611 = property on="Supprimer segment" class="Bool"("Disabled"=w885) -> ()  [unwired: 2 in, 2 out]
                        n612 = property on="Onglet_segments" class="Onglet (strict)"("Disabled"=w885) -> ()  [unwired: 2 in, 2 out]
                        n613 = property on="Insérer segment" class="Bool"("Disabled"=w885) -> ()  [unwired: 2 in, 2 out]
                        n614 = property on="Sauvegarder" class="Bool"("Disabled"=w885) -> ()  [unwired: 2 in, 2 out]
                        n615 = property on="Visualiser le profil" class="Bool"("Disabled"=w885) -> ()  [unwired: 2 in, 2 out]
                        n616 = property on="Segment à éditer/supprimer" class="NumNb (strict)"("Disabled"=w885) -> ()  [unwired: 2 in, 2 out]
                      }
                    }
                    n617 = call "Generer_listing_alarmes.vi"("Configuration"=w859) -> ("Listing alarmes"=w860:string)
                    n618 = call "Generer_listing.vi"("Listing_entrée"=w860, "Numéro de programme"=w856, "Programme"=w855) -> ("Listing_sortie"=w854:string)
                    n619 = case shown="\"Prog 1\", Par défaut" w853 {
                      tunnel: w855 -> [w865 w867 w868 w871 w873 w874 w876 w879 w881 w883]
                      tunnel: w854 -> [w864 w866 w869 w870 w872 w875 w877 w878 w880 w882]
                      frame "Prog 1", Default {
                        n620 = local write "Listing programme 1"(w864) -> ()
                        n621 = local write "Programme 1"(w865) -> ()
                      }
                      frame "Prog 2" {
                        n622 = local write "Listing programme 2"(w866) -> ()
                        n623 = local write "Programme 2"(w867) -> ()
                      }
                      frame "Prog 3" {
                        n624 = local write "Listing programme 3"(w869) -> ()
                        n625 = local write "Programme 3"(w868) -> ()
                      }
                      frame "Prog 4" {
                        n626 = local write "Listing programme 4"(w870) -> ()
                        n627 = local write "Programme 4"(w871) -> ()
                      }
                      frame "Prog 5" {
                        n628 = local write "Listing programme 5"(w872) -> ()
                        n629 = local write "Programme 5"(w873) -> ()
                      }
                      frame "Prog 6" {
                        n630 = local write "Listing programme 6"(w875) -> ()
                        n631 = local write "Programme 6"(w874) -> ()
                      }
                      frame "Prog 7" {
                        n632 = local write "Listing programme 7"(w877) -> ()
                        n633 = local write "Programme 7"(w876) -> ()
                      }
                      frame "Prog 8" {
                        n634 = local write "Listing programme 8"(w878) -> ()
                        n635 = local write "Programme 8"(w879) -> ()
                      }
                      frame "Prog 9" {
                        n636 = local write "Listing programme 9"(w880) -> ()
                        n637 = local write "Programme 9"(w881) -> ()
                      }
                      frame "Prog 10" {
                        n638 = local write "Listing programme 10"(w882) -> ()
                        n639 = local write "Programme 10"(w883) -> ()
                      }
                    }
                  }
                }
              }
            }
          }
          event "Onglets_programmes": Value Change {
            # "Si données générales écrites\non a :\nTaille_programme >= 1\n\nAlors, on active les controles\nOn met à jour les unités"
            n640 = event-data() -> ("NewVal"=w910:T1)  [unwired: 1 in, 5 out]
            n641 = case shown="\"Prog 10\"" w910 {
              tunnel: [w933 w935 w937 w939 w941 w943 w945 w947 w949 w951] -> w906
              tunnel: [u8 1 ("Numéro de programme") u8 2 ("Numéro de programme") u8 3 ("Numéro de programme") u8 4 ("Numéro de programme") u8 5 ("Numéro de programme") u8 6 ("Numéro de programme") u8 7 ("Numéro de programme") u8 8 ("Numéro de programme") u8 9 ("Numéro de programme") u8 10 ("Numéro de programme")] -> _
              frame "Prog 1", Default {
                n642 = local read "Programme 1"() -> (w933:cluster{"chaîne":string, "Valeur":dbl}[][])
              }
              frame "Prog 2" {
                n643 = local read "Programme 2"() -> (w935:cluster{"chaîne":string, "Valeur":dbl}[][])
              }
              frame "Prog 3" {
                n644 = local read "Programme 3"() -> (w937:cluster{"chaîne":string, "Valeur":dbl}[][])
              }
              frame "Prog 4" {
                n645 = local read "Programme 4"() -> (w939:cluster{"chaîne":string, "Valeur":dbl}[][])
              }
              frame "Prog 5" {
                n646 = local read "Programme 5"() -> (w941:cluster{"chaîne":string, "Valeur":dbl}[][])
              }
              frame "Prog 6" {
                n647 = local read "Programme 6"() -> (w943:cluster{"chaîne":string, "Valeur":dbl}[][])
              }
              frame "Prog 7" {
                n648 = local read "Programme 7"() -> (w945:cluster{"chaîne":string, "Valeur":dbl}[][])
              }
              frame "Prog 8" {
                n649 = local read "Programme 8"() -> (w947:cluster{"chaîne":string, "Valeur":dbl}[][])
              }
              frame "Prog 9" {
                n650 = local read "Programme 9"() -> (w949:cluster{"chaîne":string, "Valeur":dbl}[][])
              }
              frame "Prog 10" {
                n651 = local read "Programme 10"() -> (w951:cluster{"chaîne":string, "Valeur":dbl}[][])
              }
            }
            n652 = call "Dernier_element_2D.vi"("Programme"=w906) -> ("Taille/Indice N+1"=w907:i32)  [unwired: 2 out]
            n653 = Greater Or Equal?(x=w907, y=1) -> (x >= y?=w909:bool)
            n654 = case shown="Vrai" w909 {
              tunnel: w906 -> [_ w923]
              frame False {
                w911 = u8 2 ("Désactivé")
                # "Controles desactivés"
                # "Données générales non écrites"
                n655 = property on="Modif seg" class="Bool"("Disabled"=w911) -> ()  [unwired: 2 in, 2 out]
                n656 = property on="Supprimer segment" class="Bool"("Disabled"=w911) -> ()  [unwired: 2 in, 2 out]
                n657 = property on="Ajouter segment" class="Bool"("Disabled"=w911) -> ()  [unwired: 2 in, 2 out]
                n658 = property on="Onglet_segments" class="Onglet (strict)"("Disabled"=w911) -> ()  [unwired: 2 in, 2 out]
                n659 = property on="Insérer segment" class="Bool"("Disabled"=w911) -> ()  [unwired: 2 in, 2 out]
                n660 = property on="Sauvegarder" class="Bool"("Disabled"=w911) -> ()  [unwired: 2 in, 2 out]
                n661 = property on="Visualiser le profil" class="Bool"("Disabled"=w911) -> ()  [unwired: 2 in, 2 out]
                n662 = property on="Segment à éditer/supprimer" class="NumNb (strict)"("Disabled"=w911) -> ()  [unwired: 2 in, 2 out]
              }
              frame True {
                w915 = u8 0 ("Désactivé")
                # "Controles activés"
                # "Unité de palier"
                # "Unité de rampe"
                # "Données générales écrites"
                n663 = property on="Modif seg" class="Bool"("Disabled"=w915) -> ()  [unwired: 2 in, 2 out]
                n664 = property on="Supprimer segment" class="Bool"("Disabled"=w915) -> ()  [unwired: 2 in, 2 out]
                n665 = property on="Ajouter segment" class="Bool"("Disabled"=w915) -> ()  [unwired: 2 in, 2 out]
                n666 = property on="Onglet_segments" class="Onglet (strict)"("Disabled"=w915) -> ()  [unwired: 2 in, 2 out]
                n667 = Index Array(array=w923, index (row)=0 ("indice (ligne)")) -> (element=w921:cluster{"chaîne":string, "Valeur":dbl}[])  [unwired: 1 in]
                n668 = Index Array(array=w921) -> (element #1=w919:cluster{"chaîne":string, "Valeur":dbl}, element #2=w920:cluster{"chaîne":string, "Valeur":dbl})  [unwired: 2 in]
                n669 = Unbundle(w919) -> ("Valeur"=w918:dbl)  [unwired: 1 out]
                n670 = Unbundle(w920) -> ("Valeur"=w917:dbl)  [unwired: 1 out]
                n671 = property on="Insérer segment" class="Bool"("Disabled"=w915) -> ()  [unwired: 2 in, 2 out]
                n672 = property on="Sauvegarder" class="Bool"("Disabled"=w915) -> ()  [unwired: 2 in, 2 out]
                n673 = property on="Visualiser le profil" class="Bool"("Disabled"=w915) -> ()  [unwired: 2 in, 2 out]
                n674 = property on="Segment à éditer/supprimer" class="NumNb (strict)"("Disabled"=w915) -> ()  [unwired: 2 in, 2 out]
                n675 = case shown="1" w918 {
                  tunnel: ["Seconde" "Minute" "Heure"] -> w914
                  frame 0, Default {
                  }
                  frame 1 {
                  }
                  frame 2 {
                  }
                }
                n676 = case shown="1" w917 {
                  tunnel: ["Seconde(s)" "Minute(s)" "Heure(s)"] -> w916
                  frame 0, Default {
                  }
                  frame 1 {
                  }
                  frame 2 {
                  }
                }
                n677 = local write "Indicateur_Unité de palier"(w916) -> ()
                n678 = Concatenate Strings("°C/" ("chaîne"), w914) -> (w924:string)
                n679 = Concatenate Strings(w914, "(s)" ("chaîne")) -> (w912:string)
                n680 = local write "Indicateur_Unité de rampe 2"(w924) -> ()
                n681 = local write "Indicateur_Unité de rampe 1"(w912) -> ()
              }
            }
          }
          event "COM régulateur": Value Change {
            n682 = event-data() -> ()  [unwired: 1 in, 6 out]
            n683 = global read "Variables glob EUROTHERM.vi" "Nb reg dispo"() -> (w954:u8[])
            n684 = Index Array(array=w954, index="COM régulateur") -> (element=w952:u8)
            n685 = property on="Num_reg" class="NumNb (strict)"("Maximum"=w952) -> ()  [unwired: 2 in, 2 out]
          }
          event "Visualiser le profil", "Début du profil": Value Change {
            w983 = 0.0 ("cas vrai")
            w984 = 2.0 ("cas faux")
            # "Bornes du profil"
            # "Allumage et activation des voyants"
            # "Affichage et activation des courbes"
            # "Valeur initiale"
            n686 = event-data() -> ()  [unwired: 1 in, 6 out]
            n687 = global read "Variables glob EUROTHERM.vi" "Ports COM REG dispo"() -> (w963:refnum<visa-resource-name>[])
            n688 = local read "COM régulateur"() -> (w962:u16)
            n689 = local read "Onglet_Tinit"() -> (w968:enum32{"Définir Tinit", "Acquérir Tinit"})
            n690 = Index Array(array=w963, index=w962) -> (element=w961:refnum<visa-resource-name>)
            n691 = call "Val Tinit.vi"("Port COM run 1 REG"=w961, "Adresse"="Num_reg", "Onglet_Tinit"=w968, "Val T ini"="Val_Tinit") -> ("Température"=w969:dbl)
            n692 = local read "Programme 1"() -> (w1007:cluster{"chaîne":string, "Valeur":dbl}[][])
            n693 = local read "Programme 2"() -> (w1006:cluster{"chaîne":string, "Valeur":dbl}[][])
            n694 = local read "Programme 3"() -> (w1005:cluster{"chaîne":string, "Valeur":dbl}[][])
            n695 = local read "Programme 4"() -> (w1004:cluster{"chaîne":string, "Valeur":dbl}[][])
            n696 = local read "Programme 5"() -> (w960:cluster{"chaîne":string, "Valeur":dbl}[][])
            n697 = local read "Programme 6"() -> (w959:cluster{"chaîne":string, "Valeur":dbl}[][])
            n698 = local read "Programme 7"() -> (w958:cluster{"chaîne":string, "Valeur":dbl}[][])
            n699 = local read "Programme 8"() -> (w957:cluster{"chaîne":string, "Valeur":dbl}[][])
            n700 = local read "Programme 9"() -> (w956:cluster{"chaîne":string, "Valeur":dbl}[][])
            n701 = local read "Programme 10"() -> (w955:cluster{"chaîne":string, "Valeur":dbl}[][])
            n702 = Bundle By Name(cluster=T6 {"fractional second"=0.0, "second"=0, "minute"=0, "hour"=0, "day of month"=0, "month"=0, "year"=0, "day of week"=0, "day of year"=0, "DST"=0} ("cluster date/heure"), "hour"=1) -> (w981:T6)
            n703 = local read "Configuration"() -> (w1000:cluster{"Command (PV)":string, dbl}[])
            n704 = local read "Début du profil"() -> (w977:timestamp)
            n705 = Date/Time To Seconds(2:w981) -> (0:w978:timestamp)  [unwired: 1 in]
            n706 = Subtract(x=w977, y=w978) -> (x-y=w980:dbl)
            n707 = Build Array(w980) -> (w998:dbl[])
            n708 = Build Array(w969) -> (w999:dbl[])
            n709 = Bundle("Configuration"=w1000, "Programme 1"=w1007, "Programme 2"=w1006, "Programme 3"=w1005, "Programme 4"=w1004, "Programme 5"=w960, "Programme 6"=w959, "Programme 7"=w958, "Programme 8"=w957, "Programme 9"=w956, "Programme 10"=w955) -> (w1003:T10)  [unwired: 1 in]
            n710 = call "Generer_profil EPC3000.vi"("Temps (s)"=w998, "Num_Prog"=u8 1, "Températures (°C)"=w999, "Programmes et config"=w1003) -> ("Temps (s)"=w1001:dbl[], "Températures (°C)"=w971:dbl[], "Evennements_sortie"=w970:T11)  [unwired: 1 in]
            n711 = call "Afficher_profil.vi"("Configuration"=w1000, "Temps (s)"=w1001, "Températures (°C)"=w971, "Evennements_entrée"=w970) -> ("Graphe XY"=→"Profil":cluster{"Y":dbl[], "Y":dbl[]}[], "Type de fin"=→"Type de fin":string, "Bornes profil"=w976:T12, "Courbes à afficher"=w997:bool[])
            n712 = Unbundle By Name(w976) -> ("Temps min"=w975:dbl, "Temps max"=w974:dbl, "Tempé. min"=w973:dbl, "Tempé. max"=w972:dbl)
            n713 = for {
              tunnel: w997 -> [w1008] mode=indexing
              i -> [w1009]
              n714 = Increment(x=w1009) -> (x+1=w1010:i32)
              n715 = stacked-sequence {
                tunnel: w1008 -> [_ w1012]
                tunnel: w1010 -> [w1011 _]
                frame #0 {
                  n716 = property on="Profil" class="GraphXY (strict)"("Active Plot"=w1011) -> ()  [unwired: 2 in, 2 out]
                }
                frame #1 {
                  n717 = property on="Profil" class="GraphXY (strict)"("Plot.Visible?"=w1012) -> ()  [unwired: 2 in, 2 out]
                }
              }
            }
            n718 = Index Array(array=w997) -> (element #3=w995:bool, element #4=w993:bool, element #5=w991:bool, element #6=w987:bool, element #7=w986:bool, element #8=w985:bool)  [unwired: 8 in, 2 out]
            n719 = property on="Profil" class="GraphXY (strict)"("XScale.Minimum"=w975, "XScale.Maximum"=w974, "YScale.Minimum"=w973, "YScale.Maximum"=w972) -> ()  [unwired: 2 in, 2 out]
            n720 = Select(t=w983, s=w985, f=w984) -> (s? t:f=w988:dbl)
            n721 = property on="Appel" class="Bool (strict)"("Value"=w985, "Disabled"=w988) -> ()  [unwired: 2 in, 2 out]
            n722 = Select(t=w983, s=w986, f=w984) -> (s? t:f=w989:dbl)
            n723 = property on="Saut" class="Bool (strict)"("Value"=w986, "Disabled"=w989) -> ()  [unwired: 2 in, 2 out]
            n724 = Select(t=w983, s=w987, f=w984) -> (s? t:f=w990:dbl)
            n725 = property on="Palier" class="Bool (strict)"("Value"=w987, "Disabled"=w990) -> ()  [unwired: 2 in, 2 out]
            n726 = Select(t=w983, s=w991, f=w984) -> (s? t:f=w992:dbl)
            n727 = property on="RT" class="Bool (strict)"("Value"=w991, "Disabled"=w992) -> ()  [unwired: 2 in, 2 out]
            n728 = Select(t=w983, s=w993, f=w984) -> (s? t:f=w994:dbl)
            n729 = property on="RV" class="Bool (strict)"("Value"=w993, "Disabled"=w994) -> ()  [unwired: 2 in, 2 out]
            n730 = Select(t=w983, s=w995, f=w984) -> (s? t:f=w996:dbl)
            n731 = property on="Fin" class="Bool (strict)"("Value"=w995, "Disabled"=w996) -> ()  [unwired: 2 in, 2 out]
          }
          event "Alarme basse", "Alarme haute": Value Change {
            n732 = event-data() -> ("CtlRef"=w1022:refnum<vi>, "OldVal"=w1021:dbl)  [unwired: 1 in, 4 out]
            n733 = local read "Listing programme 10"() -> (w1015:string)
            n734 = local read "Listing programme 1"() -> (w1029:string)
            n735 = local read "Listing programme 2"() -> (w1028:string)
            n736 = local read "Listing programme 3"() -> (w1027:string)
            n737 = local read "Listing programme 4"() -> (w1026:string)
            n738 = local read "Listing programme 5"() -> (w1020:string)
            n739 = local read "Listing programme 6"() -> (w1019:string)
            n740 = local read "Listing programme 7"() -> (w1018:string)
            n741 = local read "Listing programme 8"() -> (w1017:string)
            n742 = local read "Listing programme 9"() -> (w1016:string)
            n743 = Concatenate Strings(w1029, w1028, w1027, w1026, w1020, w1019, w1018, w1017, w1016, w1015) -> (w1025:string)
            n744 = while {
              shift-right: [w1081] -> _
              shift-left: w1025 -> [w1083]
              tunnel: [w1073] -> w1024 mode=indexing
              tunnel: "Alarme haute" -> [w1071]
              tunnel: "Alarme basse" -> [w1070]
              stop <- w1075 stop-if-true
              n745 = Match Pattern(string=w1083, regular expression=" degrés") -> (before substring=w1080:string, after substring=w1081:string, offset past match=w1077:i32)  [unwired: 1 in, 1 out]
              n746 = Less Than 0?(x=w1077) -> (x < 0?=w1075:bool)
              n747 = Match Pattern(string=w1080, regular expression="vers " ("expression régulière")) -> (after substring=w1078:string)  [unwired: 1 in, 3 out]
              n748 = Fract/Exp String To Number(string=w1078) -> (number=w1076:dbl)  [unwired: 3 in, 1 out]
              n749 = In Range and Coerce(upper limit=w1071, x=w1076, lower limit=w1070) -> (In Range?=w1074:bool)  [unwired: 1 out]
              n750 = Select(t=TRUE ("cas vrai"), s=w1075, f=w1074) -> (s? t:f=w1073:bool)
            }
            n751 = Bundle("A1", "Alarme basse"="Alarme basse") -> (w1032:cluster{string, "Alarme basse":dbl})  [unwired: 1 in]
            n752 = Bundle("A2", "Alarme haute"="Alarme haute") -> (w1031:cluster{string, "Alarme haute":dbl})  [unwired: 1 in]
            n753 = Build Array(w1032, w1031) -> (w1030:cluster{string, "Alarme haute":dbl}[])
            n754 = And Array Elements(Boolean array=w1024) -> (logical AND=w1023:bool)
            n755 = case shown="Vrai" w1023 {
              tunnel: w1030 -> [_ w1068]
              tunnel: w1022 -> [w1036 _]
              tunnel: w1021 -> [w1035 _]
              frame False {
                n756 = property class="NumNb (strict)"(reference=w1036, "Value"=w1035) -> ()  [unwired: 1 in, 2 out]
                n757 = One Button Dialog(message="Alarme incompatible avec les consignes du programme") -> ()  [unwired: 1 in, 1 out]
              }
              frame True {
                n758 = local write "Configuration"(w1068) -> ()
                n759 = call "Generer_listing_alarmes.vi"("Configuration"=w1068) -> ("Listing alarmes"=w1038:string)
                n760 = local read "Programme 10"() -> (w1043:cluster{"chaîne":string, "Valeur":dbl}[][])
                n761 = local read "Programme 7"() -> (w1050:cluster{"chaîne":string, "Valeur":dbl}[][])
                n762 = local read "Programme 8"() -> (w1049:cluster{"chaîne":string, "Valeur":dbl}[][])
                n763 = local read "Programme 9"() -> (w1044:cluster{"chaîne":string, "Valeur":dbl}[][])
                n764 = local read "Programme 5"() -> (w1056:cluster{"chaîne":string, "Valeur":dbl}[][])
                n765 = local read "Programme 2"() -> (w1067:cluster{"chaîne":string, "Valeur":dbl}[][])
                n766 = local read "Programme 3"() -> (w1062:cluster{"chaîne":string, "Valeur":dbl}[][])
                n767 = local read "Programme 4"() -> (w1061:cluster{"chaîne":string, "Valeur":dbl}[][])
                n768 = local read "Programme 6"() -> (w1055:cluster{"chaîne":string, "Valeur":dbl}[][])
                n769 = local read "Programme 1"() -> (w1040:cluster{"chaîne":string, "Valeur":dbl}[][])
                n770 = call "Generer_listing.vi"("Listing_entrée"=w1038, "Numéro de programme"=u8 10, "Programme"=w1043) -> ("Listing_sortie"=w1041:string)
                n771 = call "Generer_listing.vi"("Listing_entrée"=w1038, "Numéro de programme"=u8 7, "Programme"=w1050) -> ("Listing_sortie"=w1052:string)
                n772 = call "Generer_listing.vi"("Listing_entrée"=w1038, "Numéro de programme"=u8 8, "Programme"=w1049) -> ("Listing_sortie"=w1047:string)
                n773 = call "Generer_listing.vi"("Listing_entrée"=w1038, "Numéro de programme"=u8 9, "Programme"=w1044) -> ("Listing_sortie"=w1046:string)
                n774 = call "Generer_listing.vi"("Listing_entrée"=w1038, "Numéro de programme"=u8 5, "Programme"=w1056) -> ("Listing_sortie"=w1058:string)
                n775 = call "Generer_listing.vi"("Listing_entrée"=w1038, "Numéro de programme"=u8 2, "Programme"=w1067) -> ("Listing_sortie"=w1065:string)
                n776 = call "Generer_listing.vi"("Listing_entrée"=w1038, "Numéro de programme"=u8 3, "Programme"=w1062) -> ("Listing_sortie"=w1064:string)
                n777 = call "Generer_listing.vi"("Listing_entrée"=w1038, "Numéro de programme"=u8 4, "Programme"=w1061) -> ("Listing_sortie"=w1059:string)
                n778 = call "Generer_listing.vi"("Listing_entrée"=w1038, "Numéro de programme"=u8 6, "Programme"=w1055) -> ("Listing_sortie"=w1053:string)
                n779 = call "Generer_listing.vi"("Listing_entrée"=w1038, "Numéro de programme"=u8 1, "Programme"=w1040) -> ("Listing_sortie"=w1069:string)
                n780 = local write "Listing programme 10"(w1041) -> ()
                n781 = local write "Listing programme 7"(w1052) -> ()
                n782 = local write "Listing programme 8"(w1047) -> ()
                n783 = local write "Listing programme 9"(w1046) -> ()
                n784 = local write "Listing programme 5"(w1058) -> ()
                n785 = local write "Listing programme 2"(w1065) -> ()
                n786 = local write "Listing programme 3"(w1064) -> ()
                n787 = local write "Listing programme 4"(w1059) -> ()
                n788 = local write "Listing programme 6"(w1053) -> ()
                n789 = local write "Listing programme 1"(w1069) -> ()
              }
            }
          }
          event "Saut", "Appel", "Fin", "RV", "RT", "Palier", "A1", "A2": Value Change {
            n790 = event-data() -> ()  [unwired: 1 in, 6 out]
            n791 = Build Array("A1", "A2", "Fin", "RV", "RT", "Palier", "Saut", "Appel") -> (w1092:bool[])
            n792 = for {
              tunnel: w1092 -> [w1095] mode=indexing
              i -> [w1093]
              n793 = Increment(x=w1093) -> (x+1=w1094:i32)
              n794 = stacked-sequence {
                tunnel: w1095 -> [_ w1097]
                tunnel: w1094 -> [w1096 _]
                frame #0 {
                  n795 = property on="Profil" class="GraphXY (strict)"("Active Plot"=w1096) -> ()  [unwired: 2 in, 2 out]
                }
                frame #1 {
                  n796 = property on="Profil" class="GraphXY (strict)"("Plot.Visible?"=w1097) -> ()  [unwired: 2 in, 2 out]
                }
              }
            }
          }
        }
      }
    }
  }
